vi "GDSLvIcon_DialogUpdateClass.vi"(1 "ClassPath(FilePath/ProjectTreePath/LvCLassRef)":variant, 2 "ClassName":string, 3 "Colors":T3={"Frame"=0, "Header Text Color"=0, "Header Background"=8453954, "BodyBackgroundPublic"=16121600, "BodyBackgroundProtected"=16777215, "BodyBackgroundPrivate"=16777215, "Body Text Color"=1, "Frame thickness"=1, "ProtectedPrivateSame"=TRUE, "Icon Header Size"=0, "Font Compression"=enum."Auto", "CapitalOnly"=TRUE}, 4 "AutoUpdate":bool, 5 "error in (no error)":errorcluster, 7 "HeaderToApply (take from VIRef or /use 2D-8bit header, Ignored if not wired)":variant, 9 "LibraryIcon":T1={"LibraryIcon"="Normal", "HeaderRows(1)"=0}) -> (14 "Splitter0px":bool, 15 "WholeIconOut":u8[][](array[numeric]) format="%x", 16 "Cancelled":bool, 17 "IconPictureOut":picture, 19 "error out":errorcluster)   [LabVIEW 2020]
uses:
  <resource>/Framework/Providers/Open_GDS/ClassProviders/Common/LvIcon_class/GDSLvIcon_ColorControl.ctl
  <resource>/Framework/Providers/Open_GDS/ClassProviders/Common/LvIcon_class/GDSLvIcon_ClassColorTypes.ctl
  <resource>/Framework/Providers/Open_GDS/ClassProviders/Common/LvIcon_class/GDSLvIcon_Type.ctl
  <resource>/Framework/Providers/Open_GDS/ClassProviders/Common/LvIcon_class/subvis/GDSLvIcon_TextDataType.ctl
  <resource>/Framework/Providers/Open_GDS/ClassProviders/Common/LvIcon_class/GDSLvIcon_WordCompressionType.ctl
  <resource>/Framework/Providers/Open_GDS/ClassProviders/Common/LvIcon_class/GDSLvIcon_TextAlignment.ctl
  <vilib>/event_ctls.llb/lveventtype.ctl
  <vilib>/picture/picture.llb/imagedata.ctl
  <resource>/Framework/Providers/Open_GDS/ClassProviders/Common/LvClass_class/GDSLvClass_IconSettingsType.ctl
panel:
  in  "NoSplitter":bool
  in  "_Back":bool
  in  "_OCR":bool
  in  "_MethodIconName":string caption="Body Text"
  in  "_DeleteIcon":bool
  in  "ClassIcon":u16(ring) items=["Normal", "Actor", "Message", "Interface", "Interface-I", "-", "Biosignal", "camera", "compression", "control dial", "database2", "GlobalVariable_48", "lc_testmode", "Lock-Lock-icon", "meter2", "motor_DC", "reset2", "signalProcessing", "SolidWorksModel", "sonar", "System", "Volts", "Warning2_32", "WarningOverlay", "-", "Add Icon..."]
  in  "_ClassIcon":string caption="Library icon"
  out "_Before":picture caption="Current"
  in  "_BodyColors":string caption="Body colors"
  in  "_Frame":string caption="Frame"
  in  "_Preview":string caption="Preview"
  in  "_RandomColorGeneration":string caption="Random color generation"
  in  "_Header":string caption="Header"
  in  "_Private":T2 caption="Private"
  in  "_Protected":T2 caption="Protected"
  in  "_Public":T2 caption="Public"
  in  "_Text":T2 caption="Text"
  in  "_ProtectedPrivateSame":bool=TRUE caption="Make Protected\nsame as Private"
  in  "_Dice":cluster{"Boolean 2":bool, "Dice 2":bool}
  out "_PrivateIcon":picture caption="Private icon"
  out "_ProtectedIcon":picture caption="Protected icon"
  out "_PublicIcon":picture caption="Public icon"
  out "_ClassIcon":picture caption="Library icon"
  out "_IconPreview":picture caption="Icon Preview"
  in  "_Frame":T2 caption="Frame"
  in  "_Thickness":u8=1 caption="Thickness (pixels)" min=1 max=3 step=1
  in  "_Rows":enum16{"1 Row", "2 Rows", "3 Rows"}(ring) caption="Rows"
  in  "_FontCompression":enum16{"Auto", "On", "Off"}(ring) caption="Font Compression"
  in  "_CapitalOnly":bool=TRUE caption="Force Capital Letters"
  in  "_Height":u8=9 caption="Height (pixels)" min=5 max=19
  in  "_Text":string="Endevo" caption="Text"
  in  "_HeaderBk":T2 caption="Background"
  in  "_HeaderText":T2 caption="Text"
  out "ClassName":string
  in  "_OK":bool
  out "Message":string
  in  "_Cancel":bool
  # "Backgrounds"
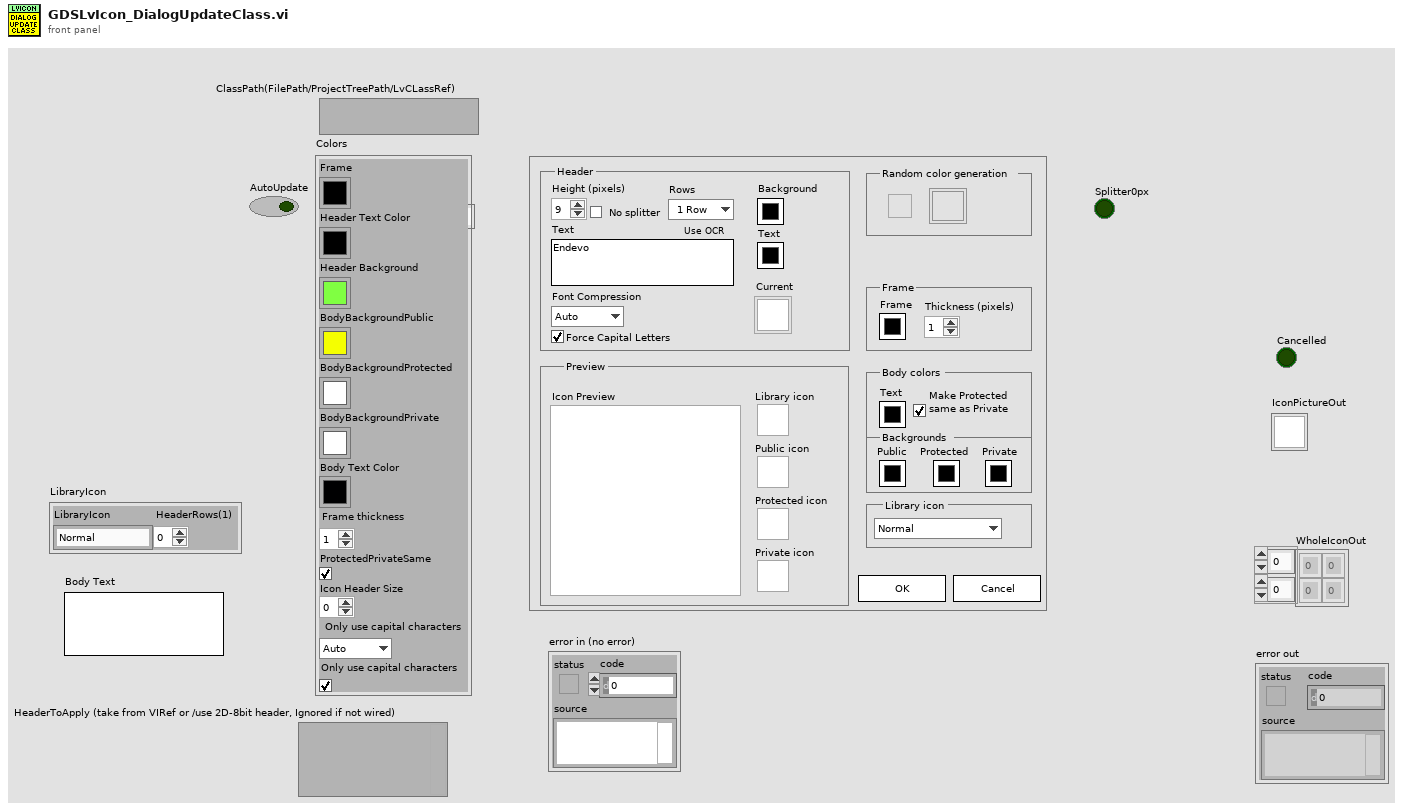
[diagram p1: front panel]
types:
  T1 = cluster{"LibraryIcon":string, "HeaderRows(1)":u8}
  T2 = typedef "GDSLvIcon_ColorControl.ctl" = cluster{"Decal":bool, "Color":u32}
  T3 = typedef "GDSLvIcon_ClassColorTypes.ctl" = cluster{"Frame":u32, "Header Text Color":u32, "Header Background":u32, "BodyBackgroundPublic":u32, "BodyBackgroundProtected":u32, "BodyBackgroundPrivate":u32, "Body Text Color":u32, "Frame thickness":u8, "ProtectedPrivateSame":bool, "Icon Header Size":u8, "Font Compression":enum16{"Auto", "On", "Off"}, "CapitalOnly":bool}
  T4 = typedef "GDSLvIcon_Type.ctl" = enum16{"LvClass", "Library", "X-Control", "LvInterface"}
  T5 = cluster{"Colors":T3, "LibraryIcon":cluster{"LibraryIcon":string, "HeaderRows(1)":u8}}
  T6 = cluster{"HText":string, "Library":refnum<vi>, "ClassItems":refnum<vi>[], "Header":u8[][], "ObjectBody":u8[][], "LvClassCreated":bool, "PreDefHeader":bool, "Type":T4, "DefaulIcons":i32, "AddIcon":i32, "NewIcon":string, "ClassBodyIcon":string, "ClassName":string, "FirstTime":bool, "_Back Colors":cluster{"_HeaderBK":u32, "_HeaderText":u32, "_Public":u32}, "IconIn":u8[][], "Cancelled":bool, "Splitter0px":bool}
  T7 = enum8{"Enabled", "Disabled", "Disabled and Grayed Out"}
  T8 = cluster{"Selection Start":u32, "Selection End":u32}
  T9 = typedef "GDSLvIcon_TextDataType.ctl" = cluster{"Text":string, "Allow Only Capital Chars":bool, "Compression":T10, "Alignment":T11}
  T10 = typedef "GDSLvIcon_WordCompressionType.ctl" = enum16{"Auto", "On", "Off"}
  T11 = typedef "GDSLvIcon_TextAlignment.ctl" = enum16{"Center", "Left", "Right"}
  T12 = typedef "lveventtype.ctl" = enum32{"Null", "Timeout", "Annotation Menu Selection", "Annotation Menu Selection?", "App Instance Close", "App Instance Close?", "Autoscale Range Change", "Bookmark Info Change", "Cell Edit", "Cell Edit?", "Cursor Grab", "Cursor Grab?", "Cursor Menu Selection", "Cursor Menu Selection?", "Cursor Move", "Cursor Release", "Data Change", "Direction Change", "Display State Change", "Drag Ended", "Drag Enter", "Drag Leave", "Drag Over", "Drag Source Update", "Drag Starting", "Drag Starting?", "Drop", "Exec State Change", "Key Down", "Key Down?", "Key Repeat", "Key Repeat?", "Key Up", "Listbox Double Click", "Menu Activation?", "Menu Selection (App)", "Menu Selection? (App)", "Menu Selection (User)", "Mouse Down", "Mouse Down?", "Mouse Enter", "Mouse Leave", "Mouse Move", "Mouse Up", "Mouse Wheel", "NI Security User Change (App)", "Pane Size", "Panel Close", "Panel Close?", "Panel Resize", "Plot Attribute Change", "Scale Range Change", "Shortcut Menu Activation?", "Shortcut Menu Selection (App)", "Shortcut Menu Selection? (App)", "Shortcut Menu Selection (User)", "Tree Double Click", "Tree Drag", "Tree Drag?", "Tree Drop", "Tree Drop?", "Tree Item Close", "Tree Item Close?", "Tree Item Open", "Tree Item Open?", "User Event", "Value Change"}
  T13 = typedef "GDSLvClass_IconSettingsType.ctl" = cluster{"Frame":u32, "Frame thickness":u8, "Header Background":u32, "Header Text":u32, "ColorPublic":u32, "ColorProtected":u32, "ColorPrivate":u32, "Body Text":u32, "ClassBodyIcon":string}
  T14 = typedef "imagedata.ctl" = cluster{"image type":i32, "image depth":i32, "image":u8[], "mask":u8[], "colors":u32[], "Rectangle":cluster{"left":i16, "top":i16, "right":i16, "bottom":i16}}
  T15 = enum32{"invalid lock state", "Not Locked", "Locked (No Password)", "Password-protected"}
  T16 = typedef "ColorControl.ctl" = cluster{"Decal":bool, "Color":u32}
  T17 = enum32{"invalid scope", "public", "private", "protected", "community"}
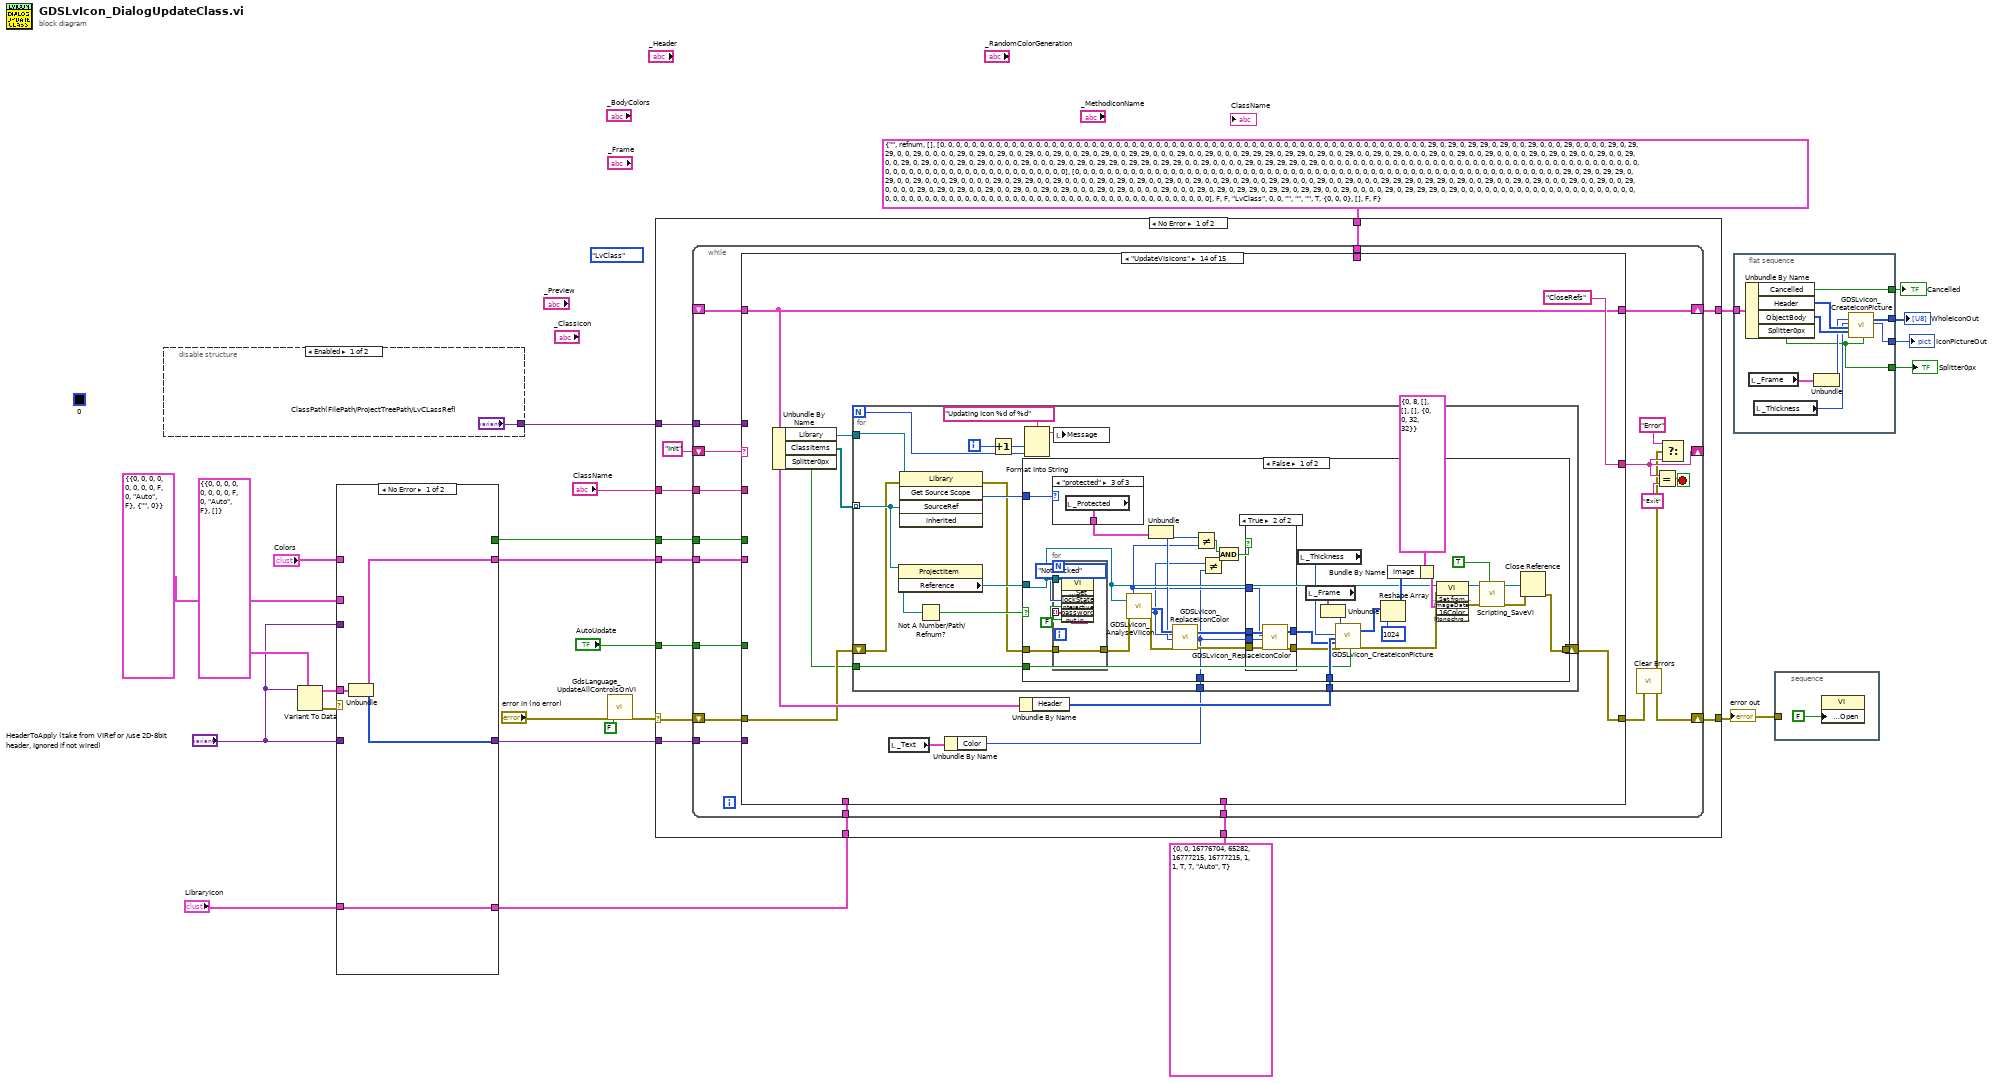
[diagram p0: block diagram]
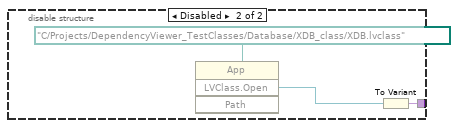
[diagram p2: hidden frame]
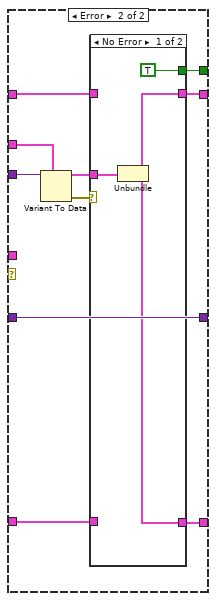
[diagram p3: hidden frame]
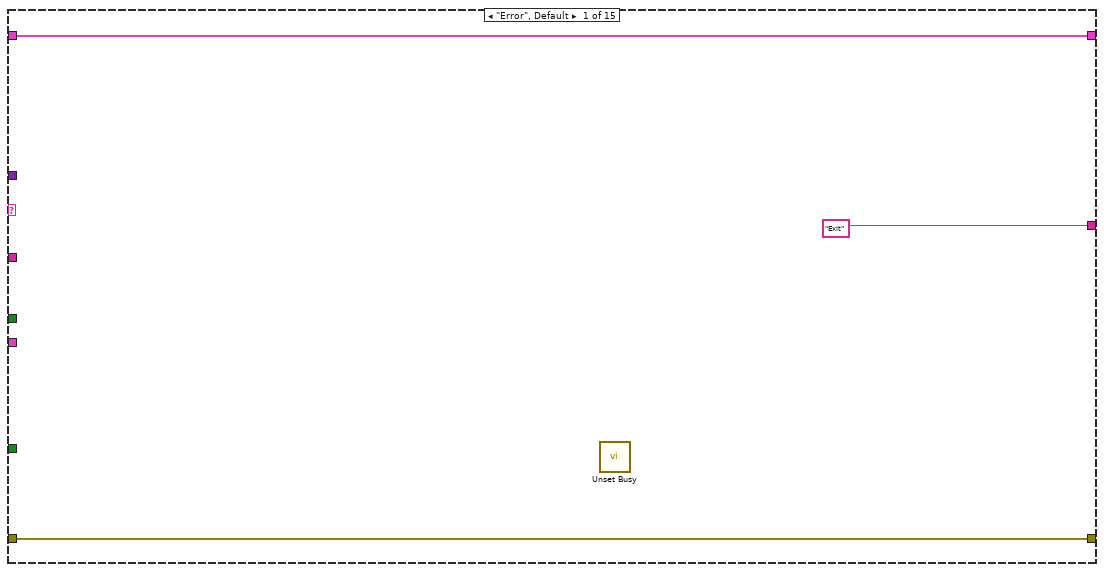
[diagram p5: hidden frame]
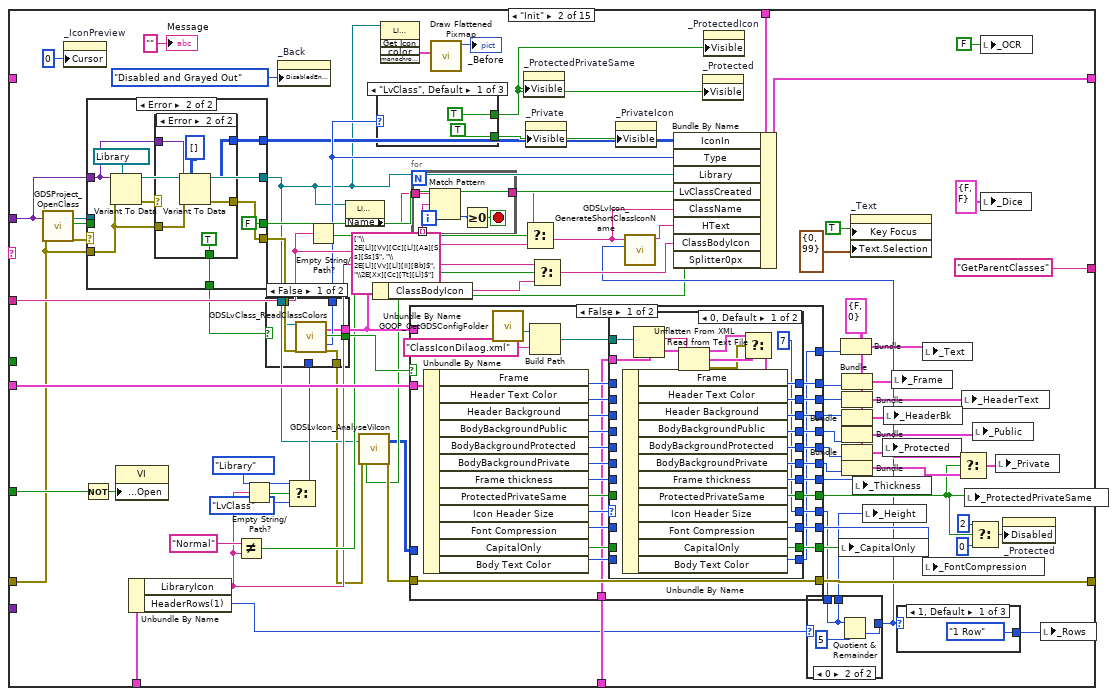
[diagram p6: hidden frame]
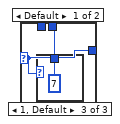
[diagram p8: hidden frame]
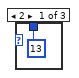
[diagram p9: hidden frame]
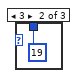
[diagram p10: hidden frame]
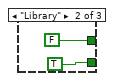
[diagram p11: hidden frame]
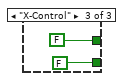
[diagram p12: hidden frame]
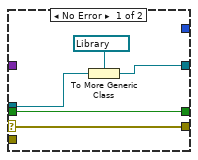
[diagram p13: hidden frame]
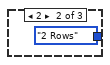
[diagram p15: hidden frame]
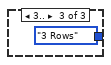
[diagram p16: hidden frame]
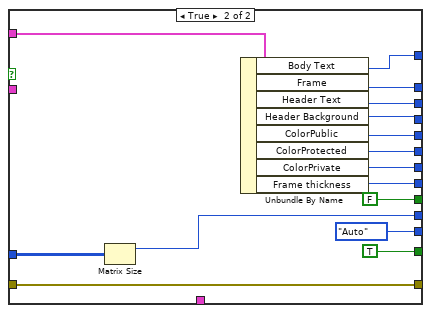
[diagram p18: hidden frame]
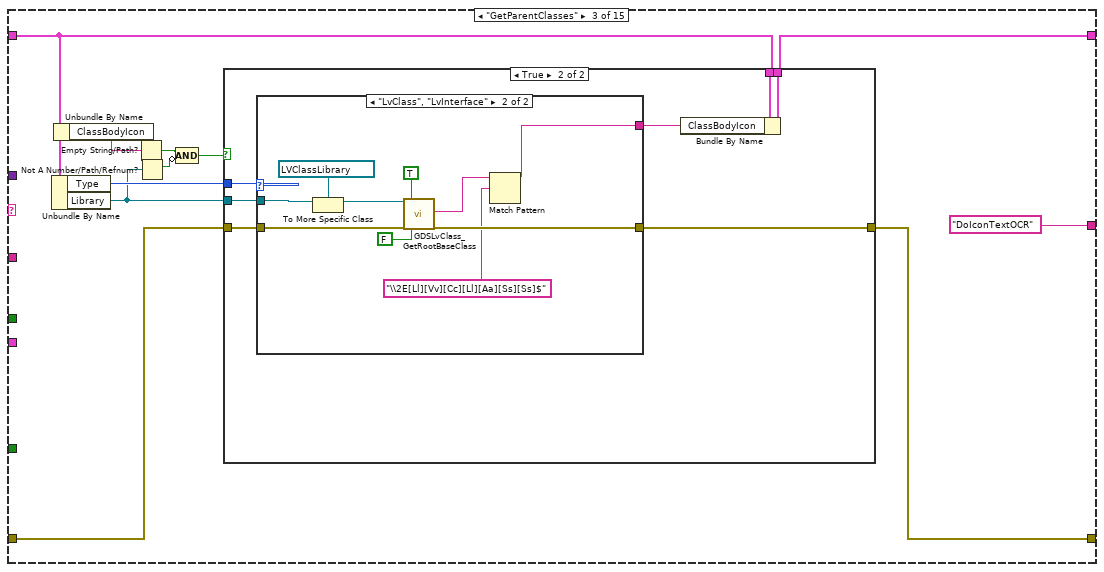
[diagram p19: hidden frame]
diagram:
  (unwired) GDSLvIcon_Type."LvClass" ("Type")
  (unwired) u32 0 ("Frame")
  n1 = disable-structure shown="Enabled" {
    disable-tunnel: ["ClassPath(FilePath/ProjectTreePath/LvCLassRef)" w29] -> w24
    frame Enabled {
    }
    frame Disabled {
      n2 = invoke class="App" method="LVClass.Open"("Path"=path "C:/Projects/DependencyViewer_TestClasses/Database/XDB_class/XDB.lvclass") -> ("LVClass.Open"=w27:refnum<vi>)  [unwired: 3 in, 3 out]
      n3 = To Variant(anything=w27) -> (Variant=w29:variant)
    }
  }
  n4 = Variant To Data(type=cluster{"Colors":T3, "TextOut":u8[][]} {"Colors"={"Frame"=0, "Header Text Color"=0, "Header Background"=0, "BodyBackgroundPublic"=0, "BodyBackgroundProtected"=0, "BodyBackgroundPrivate"=0, "Body Text Color"=0, "Frame thickness"=0, "ProtectedPrivateSame"=FALSE, "Icon Header Size"=0, "Font Compression"=enum."Auto", "CapitalOnly"=FALSE}, "TextOut"=[]} ("output cluster"), Variant="HeaderToApply (take from VIRef or /use 2D-8bit header, Ignored if not wired)") -> (data=w14:cluster{"Colors":T3, "TextOut":u8[][]}, error out=w15:errorcluster)  [unwired: 1 in]
  n5 = case shown="No Error" w15 {
    tunnel: w14 -> [w33 _]
    tunnel: [w32 w43] -> w13
    tunnel: "HeaderToApply (take from VIRef or /use 2D-8bit header, Ignored if not wired)" -> [_ w43]
    tunnel: "Colors" -> [_ w37]
    tunnel: [w31 w38] -> w11
    tunnel: "HeaderToApply (take from VIRef or /use 2D-8bit header, Ignored if not wired)" -> [_ w42]
    tunnel: T5 {"Colors"={"Frame"=0, "Header Text Color"=0, "Header Background"=0, "BodyBackgroundPublic"=0, "BodyBackgroundProtected"=0, "BodyBackgroundPrivate"=0, "Body Text Color"=0, "Frame thickness"=0, "ProtectedPrivateSame"=FALSE, "Icon Header Size"=0, "Font Compression"=enum."Auto", "CapitalOnly"=FALSE}, "LibraryIcon"={"LibraryIcon"="", "HeaderRows(1)"=0}} ("output cluster") -> [_ w41]
    tunnel: "LibraryIcon" -> [w30 w35]
    tunnel: [w30 w36] -> w7
    tunnel: [_ w34] -> w6
    frame No Error {
      n6 = Unbundle(w33) -> ("Colors"=w31:T3, "TextOut"=w32:u8[][])
    }
    frame Error {
      n7 = Variant To Data(type=w41, Variant=w42) -> (data=w39:T5, error out=w40:errorcluster)  [unwired: 1 in]
      n8 = case shown="No Error" w40 {
        tunnel: w39 -> [w47 _]
        tunnel: [w46 w49] -> w38
        tunnel: w37 -> [_ w49]
        tunnel: [w45 w48] -> w36
        tunnel: w35 -> [_ w48]
        tunnel: [TRUE _] -> w34
        frame No Error {
          n9 = Unbundle(w47) -> ("Colors"=w46:T3, "LibraryIcon"=w45:T1)
        }
        frame Error {
        }
      }
    }
  }
  n10 = call <resource>:"GdsLanguage_UpdateAllControlsOnVI.vi"("error in (no error)"="error in (no error)", "CreateLanguageFile(Use this to create a languageFile)"=FALSE) -> ("error out"=w17:errorcluster)  [unwired: 16 in, 1 out]
  n11 = case shown="No Error" w17 {
    selector: w17 -> [w61 w988]
    tunnel: [w60 w988] -> w20
    tunnel: w11 -> [w59 _]
    tunnel: "ClassName" -> [w58 _]
    tunnel: w24 -> [w57 _]
    tunnel: T6 {"HText"="", "Library"=refnum, "ClassItems"=[], "Header"=[[0, 0, 0, 0, 0, 0, 0, 0, 0, 0, 0, 0, 0, 0, 0, 0, 0, 0, 0, 0, 0, 0, 0, 0, 0, 0, 0, 0, 0, 0], [0, 0, 0, 0, 0, 0, 0, 0, 0, 0, 0, 0, 0, 0, 0, 0, 0, 0, 0, 0, 0, 0, 0, 0, 0, 0, 0, 0, 0, 0], [0, 29, 0, 29, 0, 29, 29, 0, 29, 0, 0, 29, 0, 0, 0, 29, 0, 0, 0, 0, 29, 0, 29, 29, 0, 0, 29, 0, 0, 0], [0, 29, 0, 29, 0, 29, 0, 0, 29, 0, 0, 29, 0, 0, 29, 0, 29, 0, 0, 29, 29, 0, 0, 0, 29, 0, 0, 29, 0, 0], [0, 29, 29, 29, 0, 29, 29, 0, 29, 0, 0, 29, 0, 0, 29, 0, 29, 0, 0, 0, 29, 0, 0, 29, 0, 0, 29, 0, 0, 0], [0, 29, 0, 29, 0, 29, 0, 0, 29, 0, 0, 29, 0, 0, 29, 0, 29, 0, 0, 0, 29, 0, 29, 0, 0, 0, 0, 29, 0, 0], [0, 29, 0, 29, 0, 29, 29, 0, 29, 29, 0, 29, 29, 0, 0, 29, 0, 0, 0, 0, 29, 0, 29, 29, 29, 0, 29, 0, 0, 0], [0, 0, 0, 0, 0, 0, 0, 0, 0, 0, 0, 0, 0, 0, 0, 0, 0, 0, 0, 0, 0, 0, 0, 0, 0, 0, 0, 0, 0, 0], [0, 0, 0, 0, 0, 0, 0, 0, 0, 0, 0, 0, 0, 0, 0, 0, 0, 0, 0, 0, 0, 0, 0, 0, 0, 0, 0, 0, 0, 0]], "ObjectBody"=[[0, 0, 0, 0, 0, 0, 0, 0, 0, 0, 0, 0, 0, 0, 0, 0, 0, 0, 0, 0, 0, 0, 0, 0, 0, 0, 0, 0, 0, 0], [0, 0, 0, 0, 0, 0, 0, 0, 0, 0, 0, 0, 0, 0, 0, 0, 0, 0, 0, 0, 0, 0, 0, 0, 0, 0, 0, 0, 0, 0], [0, 29, 0, 29, 0, 29, 29, 0, 29, 0, 0, 29, 0, 0, 0, 29, 0, 0, 0, 0, 29, 0, 29, 29, 0, 0, 29, 0, 0, 0], [0, 29, 0, 29, 0, 29, 0, 0, 29, 0, 0, 29, 0, 0, 29, 0, 29, 0, 0, 29, 29, 0, 0, 0, 29, 0, 0, 29, 0, 0], [0, 29, 29, 29, 0, 29, 29, 0, 29, 0, 0, 29, 0, 0, 29, 0, 29, 0, 0, 0, 29, 0, 0, 29, 0, 0, 29, 0, 0, 0], [0, 29, 0, 29, 0, 29, 0, 0, 29, 0, 0, 29, 0, 0, 29, 0, 29, 0, 0, 0, 29, 0, 29, 0, 0, 0, 0, 29, 0, 0], [0, 29, 0, 29, 0, 29, 29, 0, 29, 29, 0, 29, 29, 0, 0, 29, 0, 0, 0, 0, 29, 0, 29, 29, 29, 0, 29, 0, 0, 0], [0, 0, 0, 0, 0, 0, 0, 0, 0, 0, 0, 0, 0, 0, 0, 0, 0, 0, 0, 0, 0, 0, 0, 0, 0, 0, 0, 0, 0, 0], [0, 0, 0, 0, 0, 0, 0, 0, 0, 0, 0, 0, 0, 0, 0, 0, 0, 0, 0, 0, 0, 0, 0, 0, 0, 0, 0, 0, 0, 0]], "LvClassCreated"=FALSE, "PreDefHeader"=FALSE, "Type"=enum."LvClass", "DefaulIcons"=0, "AddIcon"=0, "NewIcon"="", "ClassBodyIcon"="", "ClassName"="", "FirstTime"=TRUE, "_Back Colors"={"_HeaderBK"=0, "_HeaderText"=0, "_Public"=0}, "IconIn"=[], "Cancelled"=FALSE, "Splitter0px"=FALSE} -> [w56 _]
    tunnel: T3 {"Frame"=0, "Header Text Color"=0, "Header Background"=16776704, "BodyBackgroundPublic"=65282, "BodyBackgroundProtected"=16777215, "BodyBackgroundPrivate"=16777215, "Body Text Color"=1, "Frame thickness"=1, "ProtectedPrivateSame"=TRUE, "Icon Header Size"=7, "Font Compression"=enum."Auto", "CapitalOnly"=TRUE} ("type") -> [w55 _]
    tunnel: "AutoUpdate" -> [w54 _]
    tunnel: w13 -> [w53 _]
    tunnel: w7 -> [w52 _]
    tunnel: w6 -> [w51 _]
    tunnel: [w50 _] -> w5
    frame No Error {
      n12 = while {
        shift-right: [w64] -> w60
        shift-left: w61 -> [w63]
        shift-right: [w65] -> _
        shift-left: "Init" -> [w68]
        shift-right: [w77] -> w50
        shift-left: _ -> [w76]
        tunnel: w59 -> [w75]
        tunnel: w58 -> [w74]
        tunnel: w57 -> [w73]
        tunnel: w56 -> [w72]
        tunnel: w55 -> [w71]
        tunnel: w54 -> [w70]
        tunnel: w53 -> [w69]
        tunnel: w52 -> [w67]
        tunnel: w51 -> [w66]
        stop <- w81 stop-if-true
        n13 = case shown="\"UpdateVIsIcons\"" w68 {
          selector: w68 -> [_ _ _ w328 w375 _ w481 _ _ w728 _ _ _ _ _]
          tunnel: w63 -> [w84 w119 w301 w334 w398 w432 w540 w557 w687 w734 w777 w785 w857 w897 w979]
          tunnel: [w84 w156 w300 w333 w398 w435 w527 w557 w687 w734 w776 w785 w847 w898 w973] -> w78
          tunnel: ["Exit" "GetParentClasses" "DoIconTextOCR" w337 "CheckPredefinedHeader" "UpdateIcons" w480 w558 w692 w727 w748 "UpdateClassDataIcon" "UpdateVIsIcons" "CloseRefs" "Exit"] -> w65
          tunnel: [w82 w157 w298 w329 w391 w434 w509 w555 w685 w724 w753 w788 w862 w900 w977] -> w77
          tunnel: w76 -> [w82 _ w299 w330 w373 w425 w488 w556 w686 w725 w753 w789 w861 w900 w977]
          tunnel: w75 -> [_ w163 _ _ _ _ _ w553 _ _ w774 _ _ _ _]
          tunnel: w74 -> [_ w154 _ _ _ _ _ _ _ _ _ _ _ _ _]
          tunnel: w73 -> [_ w122 _ _ _ _ _ _ _ _ _ _ _ _ _]
          tunnel: w72 -> [_ w158 _ _ _ _ _ _ _ _ _ _ _ _ _]
          tunnel: w71 -> [_ w150 _ _ _ _ _ _ _ _ _ _ _ _ _]
          tunnel: w70 -> [_ w149 _ _ _ _ _ w554 _ _ _ _ _ _ _]
          tunnel: w69 -> [_ _ _ _ _ w431 _ _ _ _ _ _ _ _ _]
          tunnel: w67 -> [_ w108 _ _ _ _ _ _ _ _ _ _ _ _ _]
          tunnel: w66 -> [_ _ _ _ _ _ _ w552 _ _ _ _ _ _ _]
          frame "Error", Default {
            n14 = call <vilib>:"Unset Busy.vi"() -> ()  [unwired: 11 in, 1 out]
          }
          frame "Init" {
            w135 = T2 {"Decal"=FALSE, "Color"=0} ("Frame")
            n15 = call <resource>:"GDSProject_OpenClass.vi"("ClassPath(FilePath/ProjectTreePath/LvCLassRef)"=w122, "error IO"=w119) -> ("LVClass.Open"=w118:refnum<vi>, "LvClassCreated"=w115:bool, "error out"=w121:errorcluster)  [unwired: 15 in]
            n16 = property on="_IconPreview" class="Pict"("Cursor"=0) -> ()  [unwired: 2 in, 2 out]
            n17 = Not(x=w149) -> (.not. x?=w148:bool)
            n18 = case shown="Error" w121 {
              selector: w121 -> [w197 _]
              tunnel: w122 -> [_ w200]
              tunnel: [w197 w202] -> w120
              tunnel: w119 -> [_ w201]
              tunnel: [w193 w205] -> w89
              tunnel: w118 -> [w194 _]
              tunnel: w115 -> [w196 _]
              tunnel: [w196 FALSE ("LvClassCreated")] -> w114
              tunnel: [_ w199] -> w96
              tunnel: [_ w198] -> w95
              frame No Error {
                n19 = To More Generic Class(target class=refnum<vi> refnum ("Library Refnum"), reference=w194) -> (generic class reference=w193:refnum<vi>)
              }
              frame Error {
                n20 = Variant To Data(error in=w201, type=refnum<vi> refnum ("Library Refnum"), Variant=w200) -> (data=w205:refnum<vi>, error out=w203:errorcluster)
                n21 = case shown="Error" w203 {
                  selector: w203 -> [w207 _]
                  tunnel: [w207 w210] -> w202
                  tunnel: w201 -> [_ w213]
                  tunnel: w200 -> [_ w211]
                  tunnel: [_ w209] -> w199
                  tunnel: [_ TRUE ("LvClassCreated")] -> w198
                  frame No Error {
                  }
                  frame Error {
                    n22 = Variant To Data(error in=w213, type=u8[][] [] ("TextOut"), Variant=w211) -> (data=w209:u8[][], error out=w210:errorcluster)
                  }
                }
              }
            }
            n23 = property class="VI"("Front Panel.Open"=w148) -> ()  [unwired: 2 in, 2 out]
            n24 = Unbundle By Name(w108) -> ("LibraryIcon"=w91:string, "HeaderRows(1)"=w103:u8)
            n25 = Not Equal?(x="Normal" ("LibraryIcon"), y=w91) -> (x != y?=w106:bool)
            n26 = Empty String/Path?(string/path=w91) -> (empty?=w92:bool)
            n27 = property on="_Back" class="Bool (strict)"("DisabledEnum"=T7."Disabled and Grayed Out" ("Disabled")) -> ()  [unwired: 2 in, 2 out]
            n28 = Select(t=GDSLvIcon_Type."Library" ("Type"), s=w92, f=GDSLvIcon_Type."LvClass" ("Type")) -> (s? t:f=w90:T4)
            n29 = case shown="False" w95 {
              tunnel: [w171 _] -> w151
              tunnel: w120 -> [w170 w173]
              tunnel: w89 -> [w169 _]
              tunnel: [w168 w172] -> w113
              tunnel: [w167 _] -> w109
              tunnel: [w166 w173] -> w88
              tunnel: w90 -> [_ w172]
              frame False {
                n30 = call <resource>:"GDSLvClass_ReadClassColors.vi"("Library Refnum"=w169, "error in (no error)"=w170) -> ("LvClassIconSettings"=w167:T13, "LvClassIconSettingsFound"=w171:bool, "Type"=w168:T4, "error out"=w166:errorcluster)  [unwired: 12 in, 2 out]
              }
              frame True {
              }
            }
            n31 = Empty String/Path?(string/path=w154) -> (empty?=w155:bool)
            n32 = property class="Library"(reference=w89) -> ("Name"=w111:string)  [unwired: 1 in, 2 out]
            n33 = call <resource>:"GDSLvIcon_AnalyseViIcon.vi"("ViRef/LvCLassRef/LvLibRef/ViPath/2D_Image"=w89, "error in (no error)"=w88) -> ("Splitter0px"=w86:bool, "HeaderIcon"=w85:u8[][], "error out"=w87:errorcluster)  [unwired: 4 in, 11 out]
            n34 = Unbundle By Name(w109) -> ("ClassBodyIcon"=w105:string)
            n35 = case shown="\"LvClass\", Default" w113 {
              tunnel: [TRUE FALSE FALSE] -> w116
              tunnel: [TRUE TRUE FALSE] -> w117
              frame "LvClass", Default {
              }
              frame "Library" {
              }
              frame "X-Control" {
              }
            }
            n36 = invoke class="Library" method="Get Icon"(reference=w89) -> ("color"=w123:T14)  [unwired: 4 in, 4 out]
            n37 = case shown="False" w151 {
              tunnel: [w245 w278] -> w125
              tunnel: w163 -> [w241 _]
              tunnel: [w240 w287] -> w147
              tunnel: [w239 w286] -> w139
              tunnel: [w238 w285] -> w138
              tunnel: [w237 w284] -> w137
              tunnel: [w236 w281] -> w162
              tunnel: [w235 enum16{"Auto", "On", "Off"}."Auto" ("Font Compression")] -> w161
              tunnel: [w234 TRUE ("CapitalOnly")] -> w160
              tunnel: [w223 FALSE ("ProtectedPrivateSame")] -> w129
              tunnel: [w222 w282] -> w134
              tunnel: [w221 w283] -> w136
              tunnel: w109 -> [_ w288]
              tunnel: w87 -> [w220 w277]
              tunnel: [w220 w277] -> w156
              tunnel: [w219 w280] -> w145
              tunnel: w150 -> [w217 _]
              tunnel: w85 -> [_ w279]
              frame False {
                n38 = Unbundle By Name(w241) -> ("Frame"=w233:u32, "Header Text Color"=w232:u32, "Header Background"=w231:u32, "BodyBackgroundPublic"=w230:u32, "BodyBackgroundProtected"=w229:u32, "BodyBackgroundPrivate"=w228:u32, "Frame thickness"=w227:u8, "ProtectedPrivateSame"=w226:bool, "Icon Header Size"=w246:u8, "Font Compression"=w225:enum16{"Auto", "On", "Off"}, "CapitalOnly"=w224:bool, "Body Text Color"=w218:u32)
                n39 = call <resource>:"GOOP_GetGDSConfigFolder.vi"() -> ("GDSFolderPath"=w244:path)
                n40 = Build Path(base path=w244, name or relative path="ClassIconDilaog.xml") -> (appended path=w242:path)
                n41 = case shown="0, Default" w246 {
                  selector: w246 -> [_ w276]
                  tunnel: [u8 7 ("Icon Header Size") w276] -> w245
                  tunnel: w242 -> [w264 _]
                  tunnel: [w262 w275] -> w240
                  tunnel: [w261 w274] -> w239
                  tunnel: [w260 w273] -> w238
                  tunnel: [w259 w272] -> w237
                  tunnel: [w258 w271] -> w221
                  tunnel: [w257 w270] -> w222
                  tunnel: [w256 w269] -> w236
                  tunnel: [w255 w268] -> w223
                  tunnel: [w254 w267] -> w235
                  tunnel: [w253 w266] -> w234
                  tunnel: w233 -> [_ w275]
                  tunnel: w232 -> [_ w274]
                  tunnel: w231 -> [_ w273]
                  tunnel: w230 -> [_ w272]
                  tunnel: w229 -> [_ w271]
                  tunnel: w228 -> [_ w270]
                  tunnel: w227 -> [_ w269]
                  tunnel: w226 -> [_ w268]
                  tunnel: w225 -> [_ w267]
                  tunnel: w224 -> [_ w266]
                  tunnel: w217 -> [w252 _]
                  tunnel: [w248 w265] -> w219
                  tunnel: w218 -> [_ w265]
                  frame 0, Default {
                    n42 = Read from Text File(file (use dialog)=w264) -> (text=w263:string)  [unwired: 3 in, 3 out]
                    n43 = Unflatten From XML(xml string=w263, type=w252) -> (value=w251:T3, error out=w250:errorcluster)  [unwired: 1 in]
                    n44 = Select(t=w252, s=w250, f=w251) -> (s? t:f=w249:T3)
                    n45 = Unbundle By Name(w249) -> ("Frame"=w262:u32, "Header Text Color"=w261:u32, "Header Background"=w260:u32, "BodyBackgroundPublic"=w259:u32, "BodyBackgroundProtected"=w258:u32, "BodyBackgroundPrivate"=w257:u32, "Frame thickness"=w256:u8, "ProtectedPrivateSame"=w255:bool, "Font Compression"=w254:enum16{"Auto", "On", "Off"}, "CapitalOnly"=w253:bool, "Body Text Color"=w248:u32)  [unwired: 1 out]
                  }
                  frame 1.. {
                  }
                }
              }
              frame True {
                n46 = Matrix Size(0:w279) -> (1:w278:i32)  [unwired: 1 out]
                n47 = Unbundle By Name(w288) -> ("Body Text"=w280:u32, "Frame"=w287:u32, "Header Text"=w286:u32, "Header Background"=w285:u32, "ColorPublic"=w284:u32, "ColorProtected"=w283:u32, "ColorPrivate"=w282:u32, "Frame thickness"=w281:u8)
              }
            }
            n48 = for {
              tunnel: string[] ["\\2E[Ll][Vv][Cc][Ll][Aa][Ss][Ss]$", "\\2E[Ll][Vv][Ll][Ii][Bb]$", "\\2E[Xx][Cc][Tt][Ll]$"] -> [w186] mode=indexing
              tunnel: [w183] -> w110
              tunnel: w111 -> [w182]
              stop <- w184 stop-if-true
              n49 = Match Pattern(string=w182, regular expression=w186) -> (before substring=w183:string, offset past match=w185:i32)  [unwired: 1 in, 2 out]
              n50 = Greater Or Equal To 0?(x=w185) -> (x >= 0?=w184:bool)
            }
            n51 = call <vilib>:"Draw Flattened Pixmap.vi"("image data"=w123) -> ("new picture"=→"_Before":picture)  [unwired: 8 in]
            n52 = property on="_ProtectedPrivateSame" class="Bool (strict)"("Visible"=w116) -> ()  [unwired: 2 in, 2 out]
            n53 = Select(t=w110, s=w155, f=w154) -> (s? t:f=w99:string)
            n54 = property on="_Private" class="Clust (strict)"("Visible"=w117) -> ()  [unwired: 2 in, 2 out]
            n55 = Select(t=w91, s=w106, f=w105) -> (s? t:f=w104:string)
            n56 = property on="_PrivateIcon" class="Pict"("Visible"=w117) -> ()  [unwired: 2 in, 2 out]
            n57 = property on="_Protected" class="Clust (strict)"("Visible"=w116) -> ()  [unwired: 2 in, 2 out]
            n58 = property on="_ProtectedIcon" class="Pict"("Visible"=w116) -> ()  [unwired: 2 in, 2 out]
            n59 = case shown="0" w103 {
              selector: w103 -> [w175 _]
              tunnel: [w175 w180] -> w102
              tunnel: w125 -> [_ w179]
              tunnel: [w174 w179] -> w100
              frame Default {
                n60 = case shown="1, Default" w175 {
                  tunnel: [u8 13 ("Icon Header Size") u8 19 ("Icon Header Size") u8 7 ("Icon Header Size")] -> w174
                  frame 2 {
                  }
                  frame 3 {
                  }
                  frame 1, Default {
                  }
                }
              }
              frame 0 {
                n61 = Quotient & Remainder(x=w179, y=u8 5) -> (floor(x/y)=w180:i32)  [unwired: 1 out]
              }
            }
            n62 = call <resource>:"GDSLvIcon_GenerateShortClassIconName.vi"("Rows(1)"=w102, "ClassName"=w99) -> ("ShortClassIconName"=w153:string)  [unwired: 9 in]
            n63 = Bundle By Name(cluster=w158, "IconIn"=w96, "Type"=w113, "Library"=w89, "LvClassCreated"=w114, "ClassName"=w99, "HText"=w153, "ClassBodyIcon"=w104, "Splitter0px"=w86) -> (w157:T6)
            n64 = local write "_CapitalOnly"(w160) -> ()
            n65 = Bundle(cluster=w135, "Color"=w145) -> (w144:T2)  [unwired: 1 in]
            n66 = Bundle(cluster=w135, "Color"=w147) -> (w146:T2)  [unwired: 1 in]
            n67 = Bundle(cluster=w135, "Color"=w139) -> (w143:T2)  [unwired: 1 in]
            n68 = Bundle(cluster=w135, "Color"=w138) -> (w142:T2)  [unwired: 1 in]
            n69 = Bundle(cluster=w135, "Color"=w137) -> (w141:T2)  [unwired: 1 in]
            n70 = Bundle(cluster=w135, "Color"=w136) -> (w140:T2)  [unwired: 1 in]
            n71 = Bundle(cluster=w135, "Color"=w134) -> (w133:T2)  [unwired: 1 in]
            n72 = property on="_Text" class="Str"("Key Focus"=TRUE, "Text.Selection"=T8 {"Selection Start"=0, "Selection End"=99}) -> ()  [unwired: 2 in, 2 out]
            n73 = local write "_Thickness"(w162) -> ()
            n74 = local write "_Height"(w100) -> ()
            n75 = local write "_Protected"(w140) -> ()
            n76 = local write "_HeaderBk"(w142) -> ()
            n77 = local write "_Frame"(w146) -> ()
            n78 = case shown="1, Default" w102 {
              tunnel: [enum16{"1 Row", "2 Rows", "3 Rows"}."1 Row" ("Rows") enum16{"1 Row", "2 Rows", "3 Rows"}."2 Rows" ("Rows") enum16{"1 Row", "2 Rows", "3 Rows"}."3 Rows" ("Rows")] -> w126
              frame 1, Default {
              }
              frame 2 {
              }
              frame 3.. {
              }
            }
            n79 = local write "_Text"(w144) -> ()
            n80 = local write "_FontCompression"(w161) -> ()
            n81 = Select(t=w140, s=w129, f=w133) -> (s? t:f=w159:T2)
            n82 = local write "_HeaderText"(w143) -> ()
            n83 = local write "_ProtectedPrivateSame"(w129) -> ()
            n84 = Select(t=u8 2 ("Disabled"), s=w129, f=u8 0 ("Disabled")) -> (s? t:f=w132:u8)
            n85 = local write "_Public"(w141) -> ()
            n86 = local write "_OCR"(FALSE ("_OCR")) -> ()
            n87 = local write "_Dice"(cluster{"Boolean 2":bool, "Dice":bool} {"Boolean 2"=FALSE, "Dice"=FALSE} ("Dice")) -> ()
            n88 = local write "_Private"(w159) -> ()
            n89 = property on="_Protected" class="Clust (strict)"("Disabled"=w132) -> ()  [unwired: 2 in, 2 out]
            n90 = local write "_Rows"(w126) -> ()
            "Message" <- "" ("Message")
          }
          frame "GetParentClasses" {
            n91 = Unbundle By Name(w299) -> ("Type"=w297:T4, "Library"=w293:refnum<vi>)
            n92 = Unbundle By Name(w299) -> ("ClassBodyIcon"=w296:string)
            n93 = Empty String/Path?(string/path=w296) -> (empty?=w295:bool)
            n94 = Not A Number/Path/Refnum?(number/path/refnum=w293) -> (NaN/Path/Refnum?=w294:bool)
            n95 = Compound Arithmetic op=AND(w295, invert w294) -> (w292:bool)
            n96 = case shown="True" w292 {
              tunnel: w293 -> [_ w306]
              tunnel: w301 -> [w303 w311]
              tunnel: [w303 w310] -> w300
              tunnel: w299 -> [w304 w309]
              tunnel: [w304 w308] -> w298
              tunnel: w297 -> [_ w305]
              frame False {
              }
              frame True {
                n97 = case shown="\"LvClass\", \"LvInterface\"" w305 {
                  tunnel: w306 -> [_ w315]
                  tunnel: w311 -> [w312 w322]
                  tunnel: [w312 w321] -> w310
                  tunnel: [_ w316] -> w307
                  frame Default {
                  }
                  frame "LvClass", "LvInterface" {
                    n98 = To More Specific Class(target class=refnum<vi> refnum ("LVClass.Open"), reference=w315) -> (specific class reference=w314:refnum<vi>)  [unwired: 1 in, 1 out]
                    n99 = call <resource>:"GDSLvClass_GetRootBaseClass.vi"("ViRef/Path,LvClassRef/Path"=w314, "error in (no error)"=w322, "Don'tOpenReference"=TRUE, "LimitToSpecificProviderTypeOfSameType(True)"=FALSE) -> ("ClassName"=w318:string, "error out"=w321:errorcluster)  [unwired: 9 in, 5 out]
                    n100 = Match Pattern(string=w318, regular expression="\\2E[Ll][Vv][Cc][Ll][Aa][Ss][Ss]$") -> (before substring=w316:string)  [unwired: 1 in, 3 out]
                  }
                }
                n101 = Bundle By Name(cluster=w309, "ClassBodyIcon"=w307) -> (w308:T6)
              }
            }
          }
          frame "DoIconTextOCR", "DoIconTextOCR:Idle" {
            n102 = Unbundle By Name(w330) -> ("FirstTime"=w327:bool, "ClassName"=w335:string, "HText"=w332:string, "IconIn"=w325:u8[][], "Library"=w324:refnum<vi>)  [unwired: 1 out]
            n103 = To Variant(anything=w325) -> (Variant=w323:variant)
            n104 = Not A Number/Path/Refnum?(number/path/refnum=w324) -> (NaN/Path/Refnum?=w326:bool)
            n105 = case shown="False" w326 {
              selector: w326 -> [w341 _]
              tunnel: [w348 w359] -> w336
              tunnel: w335 -> [w347 w359]
              tunnel: w334 -> [w346 w360]
              tunnel: [w345 w360] -> w333
              tunnel: w332 -> [w344 _]
              tunnel: w327 -> [w343 _]
              tunnel: w324 -> [w340 _]
              tunnel: w323 -> [w339 _]
              frame False {
                # "First Time and OCR Text Found"
                n106 = Select(t=w339, s=w341, f=w340) -> (s? t:f=w338:variant)
                n107 = call <resource>:"GDSLvIcon_AnalyseViIcon.vi"("ViRef/LvCLassRef/LvLibRef/ViPath/2D_Image"=w338, "DoATextOCR(False)"=TRUE, "error in (no error)"=w346) -> ("HeadText(OCR)"=w342:string, "error out"=w345:errorcluster)  [unwired: 3 in, 12 out]
                n108 = call <resource>:"GOOP_OCREvaluation.vi"("OcrText"=w342, "Viname"=w347) -> ("Match"=w350:bool)  [unwired: 9 in]
                n109 = Empty String/Path?(string/path=w342) -> (empty?=w353:bool)
                n110 = Compound Arithmetic op=AND(w343, invert w353) -> (w354:bool)
                n111 = local read "_OCR"() -> (w349:bool)
                n112 = And(x=w343, y=w350) -> (x .and. y?=w351:bool)
                n113 = Or(x=w351, y=w349) -> (x .or. y?=w352:bool)
                n114 = Select(t=w342, s=w352, f=w344) -> (s? t:f=w348:string)
                n115 = case shown="True" w354 {
                  tunnel: w350 -> [_ w356]
                  frame False {
                  }
                  frame True {
                    w357 = FALSE ("Boolean Text.Font:Bold")
                    n116 = property on="_OCR" class="Bool (strict)"("BoolText.FontBold"=w357, "BoolText.FontUnder"=w357, "Visible"=TRUE, "Value"=w356) -> ()  [unwired: 2 in, 2 out]
                  }
                }
              }
              frame True {
              }
            }
            n117 = local write "_Text"(w336) -> ()
            n118 = case shown="\"DoIconTextOCR:Idle\"" w328 {
              tunnel: ["UpdateIcons" "GetIcons"] -> w337
              frame "DoIconTextOCR:Idle" {
              }
              frame Default {
              }
            }
            n119 = Bundle By Name(cluster=w330, "FirstTime"=FALSE) -> (w329:T6)
          }
          frame "GetIcons", "GetIcons:AndSelect" {
            w384 = string[] ["Actor", "Message", "Interface", "Interface-I"] ("Strings []")
            n120 = call <resource>:"GOOP_GetProviderIniFilePath.vi"() -> ("ProviderMainFolder"=w388:path)  [unwired: 10 in, 1 out]
            n121 = Build Path(base path=w388, name or relative path="ClassBodyIcons") -> (appended path=w382:path)
            n122 = List Folder(path=w382) -> (filenames=w385:string[])  [unwired: 3 in, 3 out]
            n123 = for {
              shift-right: [w417] -> w383
              shift-left: w385 -> [w418]
              tunnel: w384 -> [w423] mode=indexing
              n124 = Concatenate Strings(w423, ".png" ("string")) -> (w421:string)
              n125 = To Lower Case(string=w421) -> (all lower case string=w419:string)
              n126 = To Lower Case(string=w418) -> (all lower case string=w420:string[])
              n127 = Search 1D Array(1D array=w420, element=w419) -> (index of element=w416:i32)  [unwired: 1 in]
              n128 = Delete From Array(array=w418, index=w416) -> (array with subset deleted=w417:string[])  [unwired: 1 in, 1 out]
            }
            n129 = Build Array (concatenate)("Normal", w384) -> (w386:string[])
            n130 = Equal?(x=w375, y="GetIcons:AndSelect") -> (x = y?=w371:bool)
            n131 = Unbundle By Name(w373) -> ("ClassBodyIcon"=w365:string, "NewIcon"=w372:string)
            n132 = for {
              tunnel: w383 -> [w411] mode=indexing
              tunnel: w382 -> [w410]
              shift-right: [w405] -> w379
              shift-left: string[] [] -> [w407]
              n133 = Build Path(base path=w410, name or relative path=w411) -> (appended path=w409:path)
              n134 = call <vilib>:"Get File Extension.vi"("file"=w409) -> ("filename without extension"=w406:string, "lowercase file extension"=w408:string)  [unwired: 6 in, 3 out]
              n135 = case shown="\"png\"" w408 {
                tunnel: w407 -> [w412 w415]
                tunnel: w406 -> [_ w414]
                tunnel: [w412 w413] -> w405
                frame Default {
                }
                frame "png" {
                  n136 = Build Array (concatenate)(w415, w414) -> (w413:string[])
                }
              }
            }
            n137 = To Lower Case(string=w365) -> (all lower case string=w363:string)
            n138 = Array Size(array=w379) -> (size(s)=w397:i32)
            n139 = Array Size(array=w386) -> (size(s)=w390:i32)
            n140 = Build Array (concatenate)("-", w379) -> (w394:string[])
            n141 = Greater Than 0?(x=w397) -> (x > 0?=w395:bool)
            n142 = Select(t=w394, s=w395, f=string[] []) -> (s? t:f=w381:string[])
            n143 = Build Array (concatenate)(w386, w381, string[] ["-", "Add Icon..."] ("f")) -> (w366:string[])
            n144 = Array Size(array=w366) -> (size(s)=w377:i32)
            n145 = case shown="Default" w363 {
              selector: w363 -> [_ w403]
              tunnel: w366 -> [_ w404]
              tunnel: [0 ("x") w402] -> w364
              frame "" {
              }
              frame Default {
                n146 = To Lower Case(string=w404) -> (all lower case string=w401:string[])
                n147 = Search 1D Array(1D array=w401, element=w403) -> (index of element=w402:i32)  [unwired: 1 in]
              }
            }
            n148 = Search 1D Array(1D array=w366, element=w372) -> (index of element=w370:i32)  [unwired: 1 in]
            n149 = Decrement(x=w377) -> (x-1=w376:i32)
            n150 = Select(t=w370, s=w371, f=w364) -> (s? t:f=w369:i32)
            n151 = Bundle By Name(cluster=w373, "AddIcon"=w376, "DefaulIcons"=w390) -> (w391:T6)
            n152 = Max & Min(x=0, y=w369) -> (max(x,y)=w367:i32)  [unwired: 1 out]
            n153 = Greater?(x=w367, y=w390) -> (0:w392:bool)
            n154 = property on="ClassIcon" class="Ring (strict)"("Strings []"=w366, "Value"=w367) -> ()  [unwired: 2 in, 2 out]
            n155 = property on="_DeleteIcon" class="Bool"("Visible"=w392) -> ()  [unwired: 2 in, 2 out]
          }
          frame "CheckPredefinedHeader" {
            n156 = Unbundle By Name(w425) -> ("Splitter0px"=w424:bool)
            n157 = Unbundle By Name(w425) -> ("IconIn"=w428:u8[][])
            n158 = Empty Array?(array=w428) -> (empty?=w429:bool)
            n159 = case shown="True" w429 {
              tunnel: [w439 w446] -> w437
              tunnel: [w440 w445] -> w436
              tunnel: w432 -> [w439 w444]
              tunnel: w431 -> [_ w443]
              tunnel: w428 -> [w441 _]
              tunnel: [_ TRUE ("PreDefHeader")] -> w427
              frame False {
                n160 = To Variant(anything=w441) -> (Variant=w440:variant)
              }
              frame True {
                n161 = Variant To Data(error in=w444, type=refnum<vi> refnum ("reference"), Variant=w443) -> (data=w445:refnum<vi>, error out=w446:errorcluster)
              }
            }
            n162 = case shown="No Error" w437 {
              selector: w437 -> [w467 _]
              tunnel: w436 -> [w465 _]
              tunnel: [w450 w471] -> w435
              tunnel: [w464 w474] -> w433
              tunnel: w432 -> [_ w470]
              tunnel: w431 -> [_ w473]
              tunnel: [w449 w469] -> w430
              tunnel: w427 -> [w449 _]
              tunnel: [w448 w468] -> w426
              tunnel: w424 -> [_ w468]
              frame No Error {
                w451 = T2 {"Decal"=FALSE, "Color"=0} ("Frame")
                n163 = call <resource>:"GDSLvIcon_AnalyseViIcon.vi"("ViRef/LvCLassRef/LvLibRef/ViPath/2D_Image"=w465, "error in (no error)"=w467) -> ("BodyTextColor"=w463:u32, "Splitter0px"=w448:bool, "HeaderTextColor"=w461:u32, "FrameColor"=w462:u32, "FrameThickness(1)"=w458:u32, "HeaderIcon"=w464:u8[][], "HeaderBkColor"=w460:u32, "BodyBkColor"=w459:u32, "error out"=w450:errorcluster)  [unwired: 4 in, 5 out]
                n164 = Array Size(array=w464) -> (size(s)=w466:i32[])
                n165 = Index Array(array=w466) -> (element=w457:i32)  [unwired: 1 in]
                n166 = Bundle(cluster=w451, "Color"=w463) -> (w455:T2)  [unwired: 1 in]
                n167 = Bundle(cluster=w451, "Color"=w462) -> (w456:T2)  [unwired: 1 in]
                n168 = Bundle(cluster=w451, "Color"=w461) -> (w454:T2)  [unwired: 1 in]
                n169 = Bundle(cluster=w451, "Color"=w460) -> (w453:T2)  [unwired: 1 in]
                n170 = Bundle(cluster=w451, "Color"=w459) -> (w452:T2)  [unwired: 1 in]
                n171 = local write "_Thickness"(w458) -> ()
                n172 = local write "_Height"(w457) -> ()
                n173 = local write "_HeaderBk"(w453) -> ()
                n174 = local write "_Frame"(w456) -> ()
                n175 = local write "_Text"(w455) -> ()
                n176 = local write "_HeaderText"(w454) -> ()
                n177 = local write "_Public"(w452) -> ()
              }
              frame Error {
                # "TBD"
                n178 = Variant To Data(error in=w470, type=u8[][] [] ("Header"), Variant=w473) -> (data=w474:u8[][], error out=w472:errorcluster)
                n179 = case shown="Error" w472 {
                  selector: w472 -> [w477 _]
                  tunnel: [w477 w478] -> w471
                  tunnel: w470 -> [_ w478]
                  tunnel: [TRUE ("PreDefHeader") _] -> w469
                  frame No Error {
                  }
                  frame Error {
                  }
                }
              }
            }
            n180 = Bundle By Name(cluster=w425, "Header"=w433, "PreDefHeader"=w430, "Splitter0px"=w426) -> (w434:T6)
          }
          frame "UpdateIcons", "UpdateIcons:GetClassChildren" {
            n181 = Unbundle By Name(w488) -> ("PreDefHeader"=w493:bool, "Header"=w492:u8[][], "Splitter0px"=w479:bool)  [unwired: 1 out]
            n182 = local read "_Text"() -> (w482:string)
            n183 = local read "_FontCompression"() -> (w538:enum16{"Auto", "On", "Off"})
            n184 = local read "_Frame"() -> (w506:T2)
            n185 = local read "_Thickness"() -> (w486:u8)
            n186 = local read "_CapitalOnly"() -> (w523:bool)
            n187 = local read "_Height"() -> (w530:u8)
            n188 = local read "_HeaderBk"() -> (w501:T2)
            n189 = Unbundle(w506) -> ("Color"=w507:u32)  [unwired: 1 out]
            n190 = local read "_HeaderText"() -> (w505:T2)
            n191 = local read "ClassIcon"() -> (w485:u16)
            n192 = local read "_Public"() -> (w503:T2)
            n193 = property on="ClassIcon" class="Ring (strict)"() -> ("Strings []"=w484:string[])  [unwired: 2 in, 2 out]
            n194 = case shown="\"Auto\", Default" w538 {
              tunnel: [enum16{"Auto", "On", "Off"}."Auto" ("Compression") enum16{"Auto", "On", "Off"}."Off" ("Compression") enum16{"Auto", "On", "Off"}."On" ("Compression")] -> w539
              frame "Auto", Default {
              }
              frame "Off" {
              }
              frame "On" {
              }
            }
            n195 = Bundle By Name(cluster=T9 {"Text"="", "Allow Only Capital Chars"=FALSE, "Compression"=enum."Auto", "Alignment"=enum."Center"} ("Text"), "Text"=w482, "Allow Only Capital Chars"=w523, "Compression"=w539) -> (w536:T9)
            n196 = Multiply(x=u8 2, y=w486) -> (x*y=w524:u8)
            n197 = Unbundle(w503) -> ("Color"=w502:u32)  [unwired: 1 out]
            n198 = Unbundle(w501) -> ("Color"=w500:u32)  [unwired: 1 out]
            n199 = Unbundle(w505) -> ("Color"=w504:u32)  [unwired: 1 out]
            n200 = case shown="Default" w485 {
              selector: w485 -> [_ w547]
              tunnel: w484 -> [_ w548]
              tunnel: [_ w546] -> w483
              frame 0 {
              }
              frame Default {
                n201 = Index Array(array=w548, index=w547) -> (element=w546:string)
              }
            }
            n202 = Subtract(x=32, y=w524) -> (x-y=w511:i32)
            n203 = call <resource>:"GDSLvIcon_GenerateIconText.vi"("Text"=w536, "TextPixelHeight(5-30)"=w530, "Foreground color"=w504, "Background color"=w500, "error in (no error)"=w540, "Text Pixel width(32-FrameThicknes*2))"=w511) -> ("TextOut"=w491:u8[][], "error out"=w535:errorcluster)  [unwired: 9 in, 3 out]
            n204 = local read "_Protected"() -> (w497:T2)
            n205 = local read "_Text"() -> (w499:T2)
            n206 = local read "_Private"() -> (w494:T2)
            n207 = Subtract(x=32, y=w530) -> (x-y=w534:i32)
            n208 = Select(t=w492, s=w493, f=w491) -> (s? t:f=w490:u8[][])
            n209 = Subtract(x=w534, y=w524) -> (x-y=w533:i32)
            n210 = Unbundle(w499) -> ("Color"=w498:u32)  [unwired: 1 out]
            n211 = case shown="True" w479 {
              tunnel: w533 -> [w542 w543]
              tunnel: [w541 w543] -> w510
              frame False {
                n212 = Decrement(x=w542) -> (x-1=w541:i32)
              }
              frame True {
              }
            }
            n213 = Unbundle(w497) -> ("Color"=w496:u32)  [unwired: 1 out]
            n214 = Unbundle(w494) -> ("Color"=w495:u32)  [unwired: 1 out]
            n215 = call <resource>:"GDSLvIcon_GenerateIconText.vi"("Text"=T9 {"Text"="PUBLIC", "Allow Only Capital Chars"=TRUE, "Compression"=enum."Auto", "Alignment"=enum."Center"}, "TextPixelHeight(5-30)"=w510, "Foreground color"=w498, "Background color"=w502, "Text Pixel width(32-FrameThicknes*2))"=w511) -> ("TextOut"=w521:u8[][], "error out"=w519:errorcluster)  [unwired: 10 in, 3 out]
            n216 = call <resource>:"GDSLvIcon_GenerateIconText.vi"("Text"=T9 {"Text"="PROTE-\nCTED", "Allow Only Capital Chars"=TRUE, "Compression"=enum."Auto", "Alignment"=enum."Center"}, "TextPixelHeight(5-30)"=w510, "Foreground color"=w498, "Background color"=w496, "Text Pixel width(32-FrameThicknes*2))"=w511) -> ("TextOut"=w516:u8[][], "error out"=w518:errorcluster)  [unwired: 10 in, 3 out]
            n217 = call <resource>:"GDSLvIcon_GenerateIconText.vi"("Text"=T9 {"Text"="PRIVATE", "Allow Only Capital Chars"=TRUE, "Compression"=enum."Auto", "Alignment"=enum."Center"}, "TextPixelHeight(5-30)"=w510, "Foreground color"=w498, "Background color"=w495, "Text Pixel width(32-FrameThicknes*2))"=w511) -> ("TextOut"=w489:u8[][], "error out"=w512:errorcluster)  [unwired: 10 in, 3 out]
            n218 = Unbundle By Name(w488) -> ("Type"=w487:T4)
            n219 = call <resource>:"GDSLvIcon_GenerateObjectIcon.vi"("HeaderColor"=w500, "BackgroundColor"=w502, "Height"=w510, "error in (no error)"=w535, "Type"=w487, "Width(30)"=w511, "ClassBodyIcon"=w483, "_Thickness"=w486) -> ("BodyIconOut"=w508:u8[][], "error out"=w528:errorcluster)  [unwired: 10 in]
            n220 = case shown="Default" w481 {
              tunnel: ["Idle" "GetClassChildren"] -> w480
              frame Default {
              }
              frame "UpdateIcons:GetClassChildren" {
              }
            }
            n221 = call <resource>:"GDSLvIcon_CreateIconPicture.vi"("FrameColor"=w507, "FrameThickness(1)"=w486, "HeaderIconIn"=w490, "BodyIconIn"=w508, "error in (no error)"=w528, "0px Splitter(False)"=w479) -> ("IconPictureOut"=→"_ClassIcon":picture, "LargeIconPictureOut(x6)"=→"_IconPreview":picture, "error out"=w527:errorcluster)  [unwired: 8 in, 3 out]
            n222 = call <resource>:"GDSLvIcon_CreateIconPicture.vi"("FrameColor"=w507, "FrameThickness(1)"=w486, "HeaderIconIn"=w490, "BodyIconIn"=w521, "error in (no error)"=w519, "0px Splitter(False)"=w479) -> ("IconPictureOut"=→"_PublicIcon":picture)  [unwired: 8 in, 5 out]
            n223 = call <resource>:"GDSLvIcon_CreateIconPicture.vi"("FrameColor"=w507, "FrameThickness(1)"=w486, "HeaderIconIn"=w490, "BodyIconIn"=w516, "error in (no error)"=w518, "0px Splitter(False)"=w479) -> ("IconPictureOut"=→"_ProtectedIcon":picture)  [unwired: 8 in, 5 out]
            n224 = call <resource>:"GDSLvIcon_CreateIconPicture.vi"("FrameColor"=w507, "FrameThickness(1)"=w486, "HeaderIconIn"=w490, "BodyIconIn"=w489, "error in (no error)"=w512, "0px Splitter(False)"=w479) -> ("IconPictureOut"=→"_PrivateIcon":picture)  [unwired: 8 in, 5 out]
            n225 = local write "NoSplitter"(w479) -> ()
            n226 = Bundle By Name(cluster=w488, "Header"=w490, "ObjectBody"=w508) -> (w509:T6)
          }
          frame "Idle" {
            (unwired) "Idle"
            n227 = case shown="False" w554 {
              tunnel: [w561 w682] -> w558
              tunnel: w556 -> [w560 w681]
              tunnel: [w559 w681] -> w555
              tunnel: w553 -> [_ w680]
              tunnel: w552 -> [_ w676]
              frame False {
                n228 = event shown="[19] \"_OK\": Value Change" {
                  selector: _ -> [_ _ _ _ _ _ _ _ _ _ _ _ _ _ _ _ _ _ _ _ _]
                  dyn-events: _ -> [_ _ _ _ _ _ _ _ _ _ _ _ _ _ _ _ _ _ _ _ _]
                  timeout: _ -> [_ _ _ _ _ _ _ _ _ _ _ _ _ _ _ _ _ _ _ _ _]
                  tunnel: ["Exit" "UpdateIcons" "DoIconTextOCR:Idle" "Idle" "Idle" "Idle" "Idle" "RandomColors" "UpdateIcons" w601 "GetIcons" "UpdateIcons" "Idle" "UpdateIcons" "UpdateIcons" "UpdateIcons" "UpdateIcons" "UpdateIcons" "UpdateIcons" "SaveSettings" "Exit"] -> w561
                  tunnel: w560 -> [w564 w568 w571 w575 w578 w581 w584 w586 w599 w606 w623 w624 w627 w635 w644 w647 w654 w656 w668 w669 w673]
                  tunnel: [w563 w567 w571 w575 w578 w581 w584 w586 w599 w606 w623 w624 w627 w635 w644 w647 w654 w656 w666 w669 w672] -> w559
                  event Panel Close? {
                    w562 = TRUE ("Discard?")
                    n229 = event-data() -> ()  [unwired: 1 in, 3 out]
                    n230 = Bundle By Name(cluster=w564, "Cancelled"=w562) -> (w563:T6)
                    n231 = event-data("Discard?"=w562) -> ()  [unwired: 1 in, 1 out]
                  }
                  event "_Text": Value Change; "_Text": Mouse Down {
                    n232 = event-data() -> ()  [unwired: 1 in, 1 out]
                    n233 = Bundle By Name(cluster=w568, "HText"="_Text") -> (w567:T6)
                  }
                  event "_OCR": Value Change {
                    w572 = FALSE ("Boolean Text.Font:Bold")
                    n234 = event-data() -> ()  [unwired: 1 in, 6 out]
                    n235 = property on="_OCR" class="Bool (strict)"("BoolText.FontBold"=w572, "BoolText.FontUnder"=w572) -> ()  [unwired: 2 in, 2 out]
                  }
                  event "_OCR": Mouse Enter {
                    w574 = TRUE ("Boolean Text.Font:Bold")
                    n236 = event-data() -> ()  [unwired: 1 in, 4 out]
                    n237 = property on="_OCR" class="Bool (strict)"("BoolText.FontBold"=w574, "BoolText.FontUnder"=w574) -> ()  [unwired: 2 in, 2 out]
                  }
                  event "_OCR": Mouse Leave {
                    w577 = FALSE ("Boolean Text.Font:Bold")
                    n238 = event-data() -> ()  [unwired: 1 in, 4 out]
                    n239 = property on="_OCR" class="Bool (strict)"("BoolText.FontBold"=w577, "BoolText.FontUnder"=w577) -> ()  [unwired: 2 in, 2 out]
                  }
                  event "_Dice": Mouse Enter {
                    n240 = event-data() -> ()  [unwired: 1 in, 1 out]
                    n241 = local write "_Dice"(cluster{"Boolean 2":bool, "Dice":bool} {"Boolean 2"=TRUE, "Dice"=FALSE} ("Dice")) -> ()
                  }
                  event "_Dice": Mouse Leave {
                    n242 = event-data() -> ()  [unwired: 1 in, 1 out]
                    n243 = local write "_Dice"(cluster{"Boolean 2":bool, "Dice":bool} {"Boolean 2"=FALSE, "Dice"=FALSE} ("Dice")) -> ()
                  }
                  event "_Dice": Value Change {
                    n244 = event-data() -> ()  [unwired: 1 in, 6 out]
                    n245 = local write "_Dice"(cluster{"Boolean 2":bool, "Dice":bool} {"Boolean 2"=TRUE, "Dice"=FALSE} ("Dice")) -> ()
                  }
                  event "_Back": Value Change {
                    w595 = T2 {"Decal"=FALSE, "Color"=0} ("Public")
                    n246 = event-data() -> ()  [unwired: 1 in, 6 out]
                    n247 = Unbundle By Name(w599) -> ("_Back Colors._HeaderBK"=w590:u32, "_Back Colors._HeaderText"=w588:u32, "_Back Colors._Public"=w589:u32)
                    n248 = Bundle By Name(cluster=w595, "Color"=u32 0) -> (w596:T2)
                    n249 = Bundle By Name(cluster=w595, "Color"=w590) -> (w594:T2)
                    n250 = Bundle By Name(cluster=w595, "Color"=w588) -> (w593:T2)
                    n251 = Bundle By Name(cluster=w595, "Color"=w589) -> (w592:T2)
                    n252 = property on="_Back" class="Bool (strict)"("DisabledEnum"=T7."Disabled and Grayed Out" ("Disabled")) -> ()  [unwired: 2 in, 2 out]
                    n253 = local write "_Text"(w596) -> ()
                    n254 = local write "_HeaderBk"(w594) -> ()
                    n255 = local write "_HeaderText"(w593) -> ()
                    n256 = local write "_Public"(w592) -> ()
                  }
                  event "ClassIcon": Value Change {
                    n257 = event-data() -> ("OldVal"=w600:u16)  [unwired: 1 in, 5 out]
                    n258 = Unbundle By Name(w606) -> ("DefaulIcons"=w605:i32, "AddIcon"=w604:i32)
                    n259 = Equal?(x="ClassIcon", y=w604) -> (x = y?=w602:bool)
                    n260 = case shown="False" w602 {
                      tunnel: w605 -> [w610 _]
                      tunnel: "ClassIcon" -> [w608 _]
                      tunnel: ["UpdateIcons" "AddIcon"] -> w601
                      tunnel: w600 -> [_ w611]
                      frame False {
                        n261 = Greater?(x=w608, y=w610) -> (0:w609:bool)
                        n262 = property on="_DeleteIcon" class="Bool"("Visible"=w609) -> ()  [unwired: 2 in, 2 out]
                      }
                      frame True {
                        n263 = property on="ClassIcon" class="Ring (strict)"("Value"=w611) -> ()  [unwired: 2 in, 2 out]
                      }
                    }
                  }
                  event "_DeleteIcon": Value Change {
                    n264 = event-data() -> ()  [unwired: 1 in, 1 out]
                    n265 = property on="ClassIcon" class="Ring (strict)"() -> ("Strings []"=w614:string[], "Value"=w615:u16)  [unwired: 2 in, 2 out]
                    n266 = call <resource>:"GOOP_GetProviderIniFilePath.vi"() -> ("ProviderMainFolder"=w616:path)  [unwired: 10 in, 1 out]
                    n267 = Index Array(array=w614, index=w615) -> (element=w619:string)
                    n268 = Build Path(base path=w616, name or relative path="ClassBodyIcons") -> (appended path=w621:path)
                    n269 = Concatenate Strings(w619, ".png" ("string")) -> (w620:string)
                    n270 = Build Path(base path=w621, name or relative path=w620) -> (appended path=w613:path)
                    n271 = Delete(path (use dialog)=w613) -> ()  [unwired: 4 in, 3 out]
                  }
                  event "_CapitalOnly", "_FontCompression": Value Change {
                    n272 = event-data() -> ()  [unwired: 1 in, 1 out]
                  }
                  event Mouse Enter; Mouse Leave {
                    n273 = event-data() -> ("Type"=w630:T12, "CtlRef"=w634:refnum<vi>)  [unwired: 1 in]
                    n274 = Equal?(x=w630, y=lveventtype."Mouse Enter") -> (x = y?=w628:bool)
                    n275 = property class="Clust (strict)"(reference=w634) -> (reference out=w633:refnum<vi>, "Value"=w632:T16)  [unwired: 1 in, 1 out]
                    n276 = Bundle By Name(cluster=w632, "Decal"=w628) -> (w631:T16)
                    n277 = property class="Clust (strict)"(reference=w633, "Value"=w631) -> ()  [unwired: 1 in, 2 out]
                  }
                  event Value Change {
                    n278 = event-data() -> ("NewVal"=w637:T2)  [unwired: 1 in]
                    n279 = local read "_ProtectedPrivateSame"() -> (w636:bool)
                    n280 = case shown="True" w636 {
                      tunnel: w637 -> [_ w639]
                      frame False {
                      }
                      frame True {
                        n281 = local write "_Private"(w639) -> ()
                        n282 = local write "_Protected"(w639) -> ()
                      }
                    }
                  }
                  event "_ProtectedPrivateSame": Value Change {
                    n283 = event-data() -> ()  [unwired: 1 in, 1 out]
                    n284 = local read "_Protected"() -> (w646:T2)
                    n285 = local write "_Private"(w646) -> ()
                    n286 = Select(t=u8 2 ("Disabled"), s="_ProtectedPrivateSame", f=u8 0 ("Disabled")) -> (s? t:f=w642:u8)
                    n287 = property on="_Protected" class="Clust (strict)"("Disabled"=w642) -> ()  [unwired: 2 in, 2 out]
                  }
                  event "_Rows": Value Change {
                    n288 = event-data() -> ()  [unwired: 1 in, 1 out]
                    n289 = case shown="\"1 Row\", Default" "_Rows" {
                      tunnel: [u8 7 ("Icon Header Size") u8 13 ("Icon Header Size") u8 19 ("Icon Header Size")] -> w649
                      frame "1 Row", Default {
                      }
                      frame "2 Rows" {
                      }
                      frame "3 Rows" {
                      }
                    }
                    n290 = local write "_Height"(w649) -> ()
                  }
                  event "_Thickness": Value Change {
                    n291 = event-data() -> ()  [unwired: 1 in, 1 out]
                  }
                  event "_Height": Value Change {
                    n292 = event-data() -> ()  [unwired: 1 in, 1 out]
                    n293 = Quotient & Remainder(x="_Height", y=u8 5) -> (floor(x/y)=w658:u8)  [unwired: 1 out]
                    n294 = case shown="1, Default" w658 {
                      tunnel: [enum16{"1 Row", "2 Rows", "3 Rows"}."1 Row" ("Rows") enum16{"1 Row", "2 Rows", "3 Rows"}."2 Rows" ("Rows") enum16{"1 Row", "2 Rows", "3 Rows"}."3 Rows" ("Rows")] -> w659
                      frame 1, Default {
                      }
                      frame 2 {
                      }
                      frame 3.. {
                      }
                    }
                    n295 = local write "_Rows"(w659) -> ()
                  }
                  event "NoSplitter": Value Change {
                    n296 = event-data() -> ()  [unwired: 1 in, 1 out]
                    n297 = Bundle By Name(cluster=w668, "Splitter0px"="NoSplitter") -> (w666:T6)
                  }
                  event "_OK": Value Change {
                    n298 = event-data() -> ()  [unwired: 1 in, 6 out]
                    n299 = call <vilib>:"Set Busy.vi"() -> ()  [unwired: 10 in, 2 out]
                  }
                  event "_Cancel": Value Change {
                    n300 = event-data() -> ()  [unwired: 1 in, 6 out]
                    n301 = Bundle By Name(cluster=w673, "Cancelled"="_Cancel") -> (w672:T6)
                  }
                }
              }
              frame True {
                n302 = Unbundle By Name(w680) -> ("Header Text Color"=w679:u32, "Header Background"=w678:u32)
                n303 = Equal?(x=w679, y=w678) -> (x = y?=w677:bool)
                n304 = And(x=w676, y=w677) -> (x .and. y?=w675:bool)
                n305 = case shown="False" w675 {
                  tunnel: ["RandomColors:UpdateIcons:GetClassChildren" "GetClassChildren"] -> w682
                  frame True {
                  }
                  frame False {
                  }
                }
              }
            }
          }
          frame "AddIcon" {
            n306 = call <resource>:"GOOP_GetProviderIniFilePath.vi"() -> ("ProviderMainFolder"=w689:path)  [unwired: 10 in, 1 out]
            n307 = Build Path(base path=w689, name or relative path="ClassBodyIcons") -> (appended path=w688:path)
            n308 = call "File Dialog"("prompt"="Select a PNG file to usa as a class icon.", "button label"="Add icon file", "pattern (all files)"="*.png") -> ("selected path"=w691:path, "cancelled"=w693:bool)  [unwired: 9 in, 2 out]
            n309 = case shown="False" w693 {
              tunnel: [w699 "Idle"] -> w692
              tunnel: w691 -> [w701 _]
              tunnel: w688 -> [w700 _]
              tunnel: w686 -> [w698 w715]
              tunnel: [w697 w715] -> w685
              frame False {
                n310 = Copy(10:w700, 11:w701) -> (0:w702:errorcluster)  [unwired: 3 in, 2 out]
                n311 = case shown="No Error" w702 {
                  tunnel: w701 -> [w706 w714]
                  tunnel: w700 -> [_ w711]
                  tunnel: ["GetIcons:AndSelect" "Idle"] -> w699
                  tunnel: w698 -> [w705 w708]
                  tunnel: [w704 w708] -> w697
                  frame No Error {
                    n312 = call <vilib>:"Get File Extension.vi"("file"=w706) -> ("filename without extension"=w703:string)  [unwired: 6 in, 4 out]
                    n313 = Bundle By Name(cluster=w705, "NewIcon"=w703) -> (w704:T6)
                  }
                  frame Error {
                    n314 = Strip Path(path=w714) -> (name=w713:string)  [unwired: 1 out]
                    n315 = Format Into String(format string="Error trying to copy the file: %s to this folder: %s" ("message"), w713, w711) -> (resulting string=w710:string)  [unwired: 2 in, 1 out]
                    n316 = One Button Dialog(message=w710) -> ()  [unwired: 1 in, 1 out]
                  }
                }
              }
              frame True {
              }
            }
          }
          frame "RandomColors", "RandomColors:UpdateIcons:GetClassChildren" {
            w732 = T2 {"Decal"=FALSE, "Color"=0} ("Public")
            w735 = u32[] [15007601, 14876576, 16751729, 15400704, 15507711, 16775072, 12713864, 12124142, 16776704, 16754080, 16752888, 16383904, 7667498, 16754986, 12112639, 3079936, 16776704, 16745561, 9341183, 16746660, 16773906, 2792191, 16762993, 5766954, 16318226, 15517125, 13290186, 10197915, 7442943, 11316396, 9743236, 16757617, 16767648, 6618880, 16711680, 16860, 16860, 16773906, 65421, 2789375, 13714175, 12827549, 10595204, 7641720, 6062466, 8025242, 11507131, 10386594, 786176, 8584960, 16318208, 16731648, 16755616, 16734715, 14399157, 16754801, 16714752, 10026888, 3524608]
            n317 = Random Number (0-1)() -> (number: 0 to 1=w743:dbl)
            n318 = Random Number (0-1)() -> (number: 0 to 1=w738:dbl)
            n319 = Array Size(array=w735) -> (size(s)=w737:i32)
            n320 = Build Array (concatenate)(w735, u32[] [10427904, 10442496, 10444544, 10452224, 10458112, 5927680, 3633920, 1351424, 35084, 40813, 16959, 19615, 1376393, 4194441, 10748084, 10420349, 7536704, 8978459, 5963776, 3882593, 4944486, 5204291, 7553536, 5263440, 4013373, 2763306, 6447714, 9540204, 6982244, 5470832, 6056066, 40848, 11010228]) -> (w741:u32[])
            n321 = Array Size(array=w741) -> (size(s)=w744:i32)
            n322 = property on="_Back" class="Bool (strict)"("DisabledEnum"=T7."Enabled" ("Disabled")) -> ()  [unwired: 2 in, 2 out]
            n323 = Multiply(x=w737, y=w738) -> (x*y=w739:dbl)
            n324 = Multiply(x=w744, y=w743) -> (x*y=w742:dbl)
            n325 = Round Toward -Infinity(1:w739) -> (0:w736:dbl)
            n326 = Round Toward -Infinity(1:w742) -> (0:w740:dbl)
            n327 = Index Array(array=w735, index=w736) -> (element=w720:u32)
            n328 = Index Array(array=w741, index=w740) -> (element=w719:u32)
            n329 = Greater?(x=w740, y=w737) -> ()  [unwired: 1 out]
            n330 = call <resource>:"GDSLvIcon_CalculateBrightness.vi"("RGB Color In"=w719) -> ("SuggestedTextColor"=w718:u32)  [unwired: 8 in, 2 out]
            n331 = feedback #1() -> (w723:u32)  [unwired: 1 in]
            n332 = feedback-in #1(w719) -> ()
            n333 = feedback #2() -> (w722:u32)  [unwired: 1 in]
            n334 = feedback-in #2(w718) -> ()
            n335 = feedback #3() -> (w721:u32)  [unwired: 1 in]
            n336 = feedback-in #3(w720) -> ()
            n337 = call <resource>:"GDSLvIcon_CalculateBrightness.vi"("RGB Color In"=w720) -> ("SuggestedTextColor"=w717:u32)  [unwired: 8 in, 2 out]
            n338 = Bundle By Name(cluster=w725, "_Back Colors._HeaderBK"=w723, "_Back Colors._HeaderText"=w722, "_Back Colors._Public"=w721) -> (w724:T6)
            n339 = case shown="Default" w728 {
              tunnel: ["UpdateIcons" "UpdateIcons:GetClassChildren"] -> w727
              frame Default {
              }
              frame "RandomColors:UpdateIcons:GetClassChildren" {
              }
            }
            n340 = Bundle By Name(cluster=w732, "Color"=w717) -> (w733:T2)
            n341 = Bundle By Name(cluster=w732, "Color"=w719) -> (w731:T2)
            n342 = Bundle By Name(cluster=w732, "Color"=w718) -> (w730:T2)
            n343 = Bundle By Name(cluster=w732, "Color"=w720) -> (w729:T2)
            n344 = local write "_HeaderBk"(w731) -> ()
            n345 = local write "_HeaderText"(w730) -> ()
            n346 = local write "_Text"(w733) -> ()
            n347 = local write "_Public"(w729) -> ()
          }
          frame "SaveSettings" {
            n348 = local read "_CapitalOnly"() -> (w769:bool)
            n349 = local read "_HeaderBk"() -> (w765:T2)
            n350 = local read "_Frame"() -> (w766:T2)
            n351 = local read "_Protected"() -> (w759:T2)
            n352 = local read "_Height"() -> (w771:u8)
            n353 = local read "_Thickness"() -> (w773:u8)
            n354 = Unbundle By Name(w765) -> ("Color"=w764:u32)
            n355 = Unbundle By Name(w759) -> ("Color"=w758:u32)
            n356 = Unbundle(w766) -> ("Color"=w767:u32)  [unwired: 1 out]
            n357 = local read "_Public"() -> (w761:T2)
            n358 = local read "_Private"() -> (w757:T2)
            n359 = local read "_FontCompression"() -> (w770:enum16{"Auto", "On", "Off"})
            n360 = local read "_HeaderText"() -> (w762:T2)
            n361 = local read "_ProtectedPrivateSame"() -> (w772:bool)
            n362 = local read "_Text"() -> (w755:T2)
            n363 = Unbundle By Name(w755) -> ("Color"=w754:u32)
            n364 = Unbundle By Name(w757) -> ("Color"=w756:u32)
            n365 = Unbundle By Name(w761) -> ("Color"=w760:u32)
            n366 = Unbundle By Name(w762) -> ("Color"=w763:u32)
            n367 = Unbundle By Name(w753) -> ("Library"=w752:refnum<vi>)
            n368 = Bundle By Name(cluster=w774, "Frame"=w767, "Header Text Color"=w763, "Header Background"=w764, "BodyBackgroundPublic"=w760, "BodyBackgroundProtected"=w758, "BodyBackgroundPrivate"=w756, "Frame thickness"=w773, "ProtectedPrivateSame"=w772, "Icon Header Size"=w771, "Font Compression"=w770, "CapitalOnly"=w769, "Body Text Color"=w754) -> (w768:T3)
            n369 = Not A Number/Path/Refnum?(number/path/refnum=w752) -> (NaN/Path/Refnum?=w751:bool)
            n370 = Flatten To XML(6:w768) -> (2:w778:string)
            n371 = call <resource>:"GOOP_GetGDSConfigFolder.vi"() -> ("GDSFolderPath"=w780:path)
            n372 = Build Path(base path=w780, name or relative path="ClassIconDilaog.xml") -> (appended path=w775:path)
            n373 = Select(t="Exit", s=w751, f="GetClassChildren") -> (s? t:f=w748:string)
            n374 = Write to Text File(file (use dialog)=w775, text=w778, error in=w777) -> (error out=w776:errorcluster)  [unwired: 1 in, 2 out]
          }
          frame "GetClassChildren" {
            n375 = Unbundle By Name(w789) -> ("Library"=w784:refnum<vi>)
            n376 = property class="Library"(reference=w784) -> ("Children[]"=w782:refnum<vi>[])  [unwired: 1 in, 2 out]
            n377 = Array Size(array=w782) -> (size(s)=w783:i32)
            n378 = Equal To 0?(x=w783) -> (x = 0?=w781:bool)
            n379 = case shown="False" w781 {
              tunnel: [w791 _] -> w787
              tunnel: w782 -> [w790 _]
              frame False {
                n380 = while {
                  shift-right: [w799] -> _
                  shift-left: w790 -> [w804]
                  shift-right: [w793] -> w791
                  shift-left: refnum<vi>[] [] -> [w794]
                  stop <- w800 stop-if-true
                  n381 = Delete From Array(array=w804, index=0) -> (deleted portion=w798:refnum<vi>, array with subset deleted=w802:refnum<vi>[])  [unwired: 1 in]
                  n382 = property class="ProjectItem"(reference=w798) -> (reference out=w796:refnum<vi>, "Type String"=w797:string)  [unwired: 1 in, 1 out]
                  n383 = case shown="\"Class Private Data\"" w797 {
                    tunnel: w796 -> [w805 w808 w813]
                    tunnel: [_ _ w815] -> w795
                    tunnel: w794 -> [w807 w810 w814]
                    tunnel: [w806 w809 w814] -> w793
                    frame Default {
                      n384 = Build Array (concatenate)(w807, w805) -> (w806:refnum<vi>[])
                    }
                    frame "Class Private Data" {
                      n385 = Build Array (concatenate)(w808, w810) -> (w809:refnum<vi>[])
                    }
                    frame "Folder" {
                      n386 = property class="ProjectItem"(reference=w813) -> (reference out=w811:refnum<vi>, error out=w812:errorcluster, "Children[]"=w815:refnum<vi>[])  [unwired: 1 in]
                      n387 = Close Reference(reference=w811, error in (no error)=w812) -> ()  [unwired: 1 out]
                    }
                  }
                  n388 = Build Array (concatenate)(w802, w795) -> (w799:refnum<vi>[])
                  n389 = Array Size(array=w799) -> (size(s)=w801:i32)
                  n390 = Equal To 0?(x=w801) -> (x = 0?=w800:bool)
                }
              }
              frame True {
              }
            }
            n391 = Bundle By Name(cluster=w789, "ClassItems"=w787) -> (w788:T6)
          }
          frame "UpdateClassDataIcon" {
            # "Updats the Icon layer info"
            n392 = Unbundle By Name(w861) -> ("Type"=w824:T4, "Library"=w822:refnum<vi>, "ClassItems"=w860:refnum<vi>[], "Header"=w818:u8[][], "ObjectBody"=w858:u8[][], "Splitter0px"=w816:bool)
            n393 = case shown="\"LvClass\"" w824 {
              tunnel: w860 -> [w865 w875]
              tunnel: [w865 w874] -> w859
              tunnel: w857 -> [w864 w873]
              tunnel: [_ w871] -> w850
              tunnel: [w864 w867] -> w830
              frame Default {
              }
              frame "LvClass" {
                n394 = Delete From Array(array=w875, index=0) -> (deleted portion=w872:refnum<vi>, array with subset deleted=w874:refnum<vi>[])  [unwired: 1 in]
                n395 = property class="ProjectItem"(reference=w872, error in=w873) -> (reference out=w870:refnum<vi>, error out=w868:errorcluster, "Reference"=w871:refnum<vi>)
                n396 = Close Reference(reference=w870, error in (no error)=w868) -> ()  [unwired: 1 out]
                n397 = call <resource>:"GDSError_ClearError.vi"("code"=1055, "error in (no error)"=w868) -> ("error out"=w867:errorcluster)  [unwired: 16 in, 1 out]
              }
            }
            n398 = case shown="\"LvClass\", Default" w824 {
              tunnel: [_ i32[] [5] ("codes")] -> w825
              tunnel: [w886 _] -> w823
              frame "LvClass", Default {
                n399 = local read "ClassIcon"() -> (w888:u16)
                n400 = property on="ClassIcon" class="Ring (strict)"() -> ("Strings []"=w887:string[])  [unwired: 2 in, 2 out]
                n401 = case shown="Default" w888 {
                  selector: w888 -> [_ w890]
                  tunnel: w887 -> [_ w891]
                  tunnel: [_ w889] -> w886
                  frame 0 {
                  }
                  frame Default {
                    n402 = Index Array(array=w891, index=w890) -> (element=w889:string)
                  }
                }
              }
              frame "X-Control" {
              }
            }
            n403 = local read "_HeaderText"() -> (w838:T2)
            n404 = local read "_Protected"() -> (w836:T2)
            n405 = local read "_Frame"() -> (w843:T2)
            n406 = local read "_Private"() -> (w839:T2)
            n407 = local read "_HeaderBk"() -> (w841:T2)
            n408 = local read "_Public"() -> (w834:T2)
            n409 = local read "_Thickness"() -> (w819:u8)
            n410 = local read "_Text"() -> (w833:T2)
            n411 = Unbundle(w843) -> ("Color"=w820:u32)  [unwired: 1 out]
            n412 = Unbundle By Name(w839) -> ("Color"=w837:u32)
            n413 = Unbundle By Name(w836) -> ("Color"=w835:u32)
            n414 = Unbundle By Name(w838) -> ("Color"=w840:u32)
            n415 = Unbundle By Name(w841) -> ("Color"=w842:u32)
            n416 = Unbundle By Name(w834) -> ("Color"=w832:u32)
            n417 = Unbundle By Name(w833) -> ("Color"=w831:u32)
            n418 = call <resource>:"GDSLvIcon_CreateIconPicture.vi"("FrameColor"=w820, "FrameThickness(1)"=w819, "HeaderIconIn"=w818, "BodyIconIn"=w858, "error in (no error)"=w830, "0px Splitter(False)"=w816) -> ("WholeIconOut"=w829:u8[][], "error out"=w821:errorcluster)  [unwired: 8 in, 4 out]
            n419 = Bundle By Name(cluster=T13 {"Frame"=0, "Frame thickness"=3, "Header Background"=8453954, "Header Text"=0, "ColorPublic"=16121600, "ColorProtected"=16777215, "ColorPrivate"=16777215, "Body Text"=0, "ClassBodyIcon"=""} ("LvClassIconSettings"), "ClassBodyIcon"=w823, "Body Text"=w831, "ColorPublic"=w832, "ColorProtected"=w835, "ColorPrivate"=w837, "Header Text"=w840, "Header Background"=w842, "Frame thickness"=w819, "Frame"=w820) -> (w844:T13)
            n420 = call <resource>:"GDSLvIcon_UpdateLibraryLayers.vi"("Library Refnum in"=w822, "FrameColor"=w820, "FrameThickness(1)"=w819, "HeaderIconIn"=w818, "error in (no error)"=w821, "0px Splitter(False)"=w816) -> ("error out"=w817:errorcluster)  [unwired: 12 in, 1 out]
            n421 = Reshape Array(w829, 1024 ("dimension size")) -> (w863:u8[])
            n422 = Bundle By Name(cluster=T14 {"image type"=0, "image depth"=8, "image"=[], "mask"=[], "colors"=[], "Rectangle"={"left"=0, "top"=0, "right"=32, "bottom"=32}} ("image data"), "image"=w863) -> (w826:T14)
            n423 = case shown="\"LvClass\"" w824 {
              tunnel: w821 -> [w876 w885]
              tunnel: [w876 w878] -> w851
              tunnel: w850 -> [_ w882]
              tunnel: w826 -> [_ w881]
              tunnel: w817 -> [_ _]
              frame Default {
              }
              frame "LvClass" {
                n424 = invoke class="VI" method="VI Icon.Set from Image Data"(reference=w882, error in=w885, "ImageData"=w881) -> (reference out=w884:refnum<vi>, error out=w883:errorcluster)  [unwired: 3 in, 4 out]
                n425 = invoke class="VI" method="Save.Instrument"(reference=w884, error in=w883) -> (reference out=w880:refnum<vi>, error out=w879:errorcluster)  [unwired: 4 in, 4 out]
                n426 = Close Reference(reference=w880) -> ()  [unwired: 1 in, 1 out]
                n427 = call <resource>:"GDSError_ClearError.vi"("code"=1055, "error in (no error)"=w879) -> ("error out"=w878:errorcluster)  [unwired: 16 in, 1 out]
              }
            }
            n428 = call <resource>:"GDSLvClass_StoreClassColors.vi"("Library Refnum"=w822, "LvClassIconSettings"=w844, "error in (no error)"=w851) -> ("Library Refnum"=w852:refnum<vi>, "error out"=w849:errorcluster)  [unwired: 15 in]
            n429 = Bundle By Name(cluster=w861, "ClassItems"=w859) -> (w862:T6)
            n430 = invoke class="Library" method="Set Icon"(reference=w852, error in=w849, "color"=w826) -> (reference out=w855:refnum<vi>, error out=w854:errorcluster)  [unwired: 2 in, 3 out]
            n431 = stacked-sequence {
              tunnel: w851 -> [_]
              frame #0 {
                n432 = local write "Message"("Updating Class template" ("Message")) -> ()
              }
            }
            n433 = invoke class="Library" method="Save"(reference=w855, error in=w854) -> (error out=w848:errorcluster)  [unwired: 2 in, 3 out]
            n434 = local write "Message"("Updating Object Icon" ("Message")) -> ()
            n435 = call <resource>:"GDSError_ClearError.vi"("code"=1055, "codes"=w825, "error in (no error)"=w848) -> ("error out"=w847:errorcluster)  [unwired: 15 in, 1 out]
          }
          frame "UpdateVIsIcons" {
            n436 = Unbundle By Name(w900) -> ("Library"=w901:refnum<vi>, "ClassItems"=w903:refnum<vi>[], "Splitter0px"=w894:bool)
            n437 = local read "_Text"() -> (w896:T2)
            n438 = Unbundle By Name(w896) -> ("Color"=w895:u32)
            n439 = Unbundle By Name(w900) -> ("Header"=w899:u8[][])
            n440 = for {
              N -> [w906]
              tunnel: w903 -> [w918] mode=indexing
              tunnel: w901 -> [w919]
              shift-right: [w912] -> w898
              shift-left: w897 -> [w913]
              tunnel: w899 -> [w911]
              tunnel: w895 -> [w905]
              tunnel: w894 -> [w904]
              i -> [w910]
              n441 = property class="ProjectItem"(reference=w918) -> ("Reference"=w916:refnum<vi>)  [unwired: 1 in, 2 out]
              n442 = invoke class="Library" method="Get Source Scope"(reference=w919, error in=w913, "SourceRef"=w918) -> (error out=w914:errorcluster, "GetSourceScope"=w915:T17)  [unwired: 2 in, 3 out]
              n443 = Not A Number/Path/Refnum?(number/path/refnum=w916) -> (NaN/Path/Refnum?=w917:bool)
              n444 = Increment(x=w910) -> (x+1=w909:i32)
              n445 = case shown="False" w917 {
                tunnel: w916 -> [w942 _]
                tunnel: w915 -> [w954 _]
                tunnel: w914 -> [w941 w972]
                tunnel: [w952 w972] -> w912
                tunnel: w911 -> [w951 _]
                tunnel: w905 -> [w922 _]
                tunnel: w904 -> [w924 _]
                frame False {
                  n446 = for {
                    tunnel: w942 -> [w966]
                    tunnel: string[] ["goop rules", "i love goteborg", "Endevo Knows Goop!"] -> [w965] mode=indexing
                    tunnel: w941 -> [w964]
                    tunnel: [w964] -> w940
                    w967 = FALSE ("Interactive")
                    n447 = invoke class="VI" method="Lock State.Set"(reference=w966, "lockState"=T15."Not Locked" ("Lock State"), "interactive"=w967, "password"=w965, "put in Cache"=w967) -> ()  [unwired: 2 in, 7 out]
                  }
                  n448 = case shown="\"protected\"" w954 {
                    tunnel: [w969 w970 w971] -> w934
                    frame "public", Default {
                      n449 = local read "_Public"() -> (w969:T2)
                    }
                    frame "private" {
                      n450 = local read "_Private"() -> (w970:T2)
                    }
                    frame "protected" {
                      n451 = local read "_Protected"() -> (w971:T2)
                    }
                  }
                  n452 = call <resource>:"GDSLvIcon_AnalyseViIcon.vi"("ViRef/LvCLassRef/LvLibRef/ViPath/2D_Image"=w942, "error in (no error)"=w940) -> ("BodyTextColor"=w925:u32, "BodyIcon"=w955:u8[][], "BodyBkColor"=w921:u32, "error out"=w953:errorcluster)  [unwired: 4 in, 10 out]
                  n453 = Unbundle(w934) -> ("Color"=w931:u32)  [unwired: 1 out]
                  n454 = call <resource>:"GDSLvIcon_ReplaceIconColor.vi"("IconIn"=w955, "OldColor"=w921, "NewColor"=w931, "error in (no error)"=w953) -> ("IconOut"=w929:u8[][], "error out"=w927:errorcluster)  [unwired: 14 in]
                  n455 = Not Equal?(x=w931, y=w925) -> (x != y?=w930:bool)
                  n456 = Not Equal?(x=w921, y=w922) -> (x != y?=w920:bool)
                  n457 = And(x=w930, y=w920) -> (x .and. y?=w923:bool)
                  n458 = case shown="True" w923 {
                    tunnel: w929 -> [w957 w963]
                    tunnel: [w957 w962] -> w928
                    tunnel: w927 -> [w956 w961]
                    tunnel: [w956 w960] -> w926
                    tunnel: w922 -> [_ w959]
                    tunnel: w925 -> [_ w958]
                    frame False {
                    }
                    frame True {
                      n459 = call <resource>:"GDSLvIcon_ReplaceIconColor.vi"("IconIn"=w963, "OldColor"=w958, "NewColor"=w959, "error in (no error)"=w961) -> ("IconOut"=w962:u8[][], "error out"=w960:errorcluster)  [unwired: 14 in]
                    }
                  }
                  n460 = local read "_Thickness"() -> (w944:u8)
                  n461 = local read "_Frame"() -> (w933:T2)
                  n462 = Unbundle(w933) -> ("Color"=w935:u32)  [unwired: 1 out]
                  n463 = call <resource>:"GDSLvIcon_CreateIconPicture.vi"("FrameColor"=w935, "FrameThickness(1)"=w944, "HeaderIconIn"=w951, "BodyIconIn"=w928, "error in (no error)"=w926, "0px Splitter(False)"=w924) -> ("WholeIconOut"=w948:u8[][], "error out"=w945:errorcluster)  [unwired: 8 in, 4 out]
                  n464 = Reshape Array(w948, 1024 ("dimension size")) -> (w946:u8[])
                  n465 = Bundle By Name(cluster=T14 {"image type"=0, "image depth"=8, "image"=[], "mask"=[], "colors"=[], "Rectangle"={"left"=0, "top"=0, "right"=32, "bottom"=32}} ("image data"), "image"=w946) -> (w949:T14)
                  n466 = invoke class="VI" method="VI Icon.Set from Image Data"(reference=w942, error in=w945, "ImageData"=w949) -> (reference out=w938:refnum<vi>, error out=w939:errorcluster)  [unwired: 3 in, 4 out]
                  n467 = call <resource>:"Scripting_SaveVi.vi"("ForceResaving(False)"=TRUE, "error in (no error)"=w939, "VIRefToSaveIn"=w938) -> ("error out"=w936:errorcluster, "VIRefToSaveOut"=w937:refnum<vi>)  [unwired: 7 in]
                  n468 = Close Reference(reference=w937, error in (no error)=w936) -> (error out=w952:errorcluster)
                }
                frame True {
                }
              }
              n469 = Format Into String(format string="Updating Icon %d of %d", w909, w906) -> (resulting string=w907:string)  [unwired: 2 in, 1 out]
              n470 = local write "Message"(w907) -> ()
            }
          }
          frame "CloseRefs" {
            n471 = Unbundle By Name(w977) -> ("LvClassCreated"=w975:bool, "Library"=w981:refnum<vi>, "ClassItems"=w980:refnum<vi>[])
            n472 = Close Reference(reference=w980, error in (no error)=w979) -> (error out=w978:errorcluster)
            n473 = case shown="True" w975 {
              tunnel: w981 -> [_ w987]
              tunnel: w978 -> [w984 w986]
              tunnel: [w984 w985] -> w974
              frame False {
              }
              frame True {
                n474 = Close Reference(reference=w987, error in (no error)=w986) -> (error out=w985:errorcluster)
              }
            }
            n475 = stacked-sequence {
              tunnel: w974 -> [w982]
              tunnel: [w983] -> _
              tunnel: [w982] -> w973
              frame #0 {
                n476 = call <vilib>:"Unset Busy.vi"("error in (no error)"=w982) -> ("error out"=w983:errorcluster)  [unwired: 10 in]
              }
            }
          }
        }
        n477 = call <vilib>:"Clear Errors.vi"("error in (no error)"=w78) -> ("error out"=w64:errorcluster)  [unwired: 5 in, 1 out]
        n478 = Equal?(x=w65, y="Exit") -> (x = y?=w81:bool)
        n479 = Select(t="Error", s=w64, f=w65) -> ()  [unwired: 1 out]
      }
    }
    frame Error {
    }
  }
  "error out" <- w20
  n480 = flat-sequence {
    tunnel: w5 -> [w998]
    tunnel: [w997] -> w4
    tunnel: [w991] -> w3
    tunnel: [w990] -> w2
    tunnel: [w989] -> w1
    frame #0 {
      n481 = Unbundle By Name(w998) -> ("Cancelled"=w997:bool, "Header"=w996:u8[][], "ObjectBody"=w995:u8[][], "Splitter0px"=w989:bool)
      n482 = local read "_Frame"() -> (w994:T2)
      n483 = local read "_Thickness"() -> (w993:u8)
      n484 = Unbundle(w994) -> ("Color"=w992:u32)  [unwired: 1 out]
      n485 = call <resource>:"GDSLvIcon_CreateIconPicture.vi"("FrameColor"=w992, "FrameThickness(1)"=w993, "HeaderIconIn"=w996, "BodyIconIn"=w995, "0px Splitter(False)"=w989) -> ("WholeIconOut"=w991:u8[][], "IconPictureOut"=w990:picture)  [unwired: 9 in, 4 out]
    }
  }
  n486 = stacked-sequence {
    tunnel: w20 -> [_]
    frame #0 {
      n487 = property class="VI"("Front Panel.Open"=FALSE ("Front Panel Window:Open")) -> ()  [unwired: 2 in, 2 out]
    }
  }
  "Cancelled" <- w4
  "WholeIconOut" <- w3
  "IconPictureOut" <- w2
  "Splitter0px" <- w1
